vi "Consumer.vi"(8 "error in (no error)":errorcluster, 9 "Data":variant, 10 "Case ID":string, 11 "Monkey in":refnum<class "Monkey.lvclass">) -> (0 "error out":errorcluster, 3 "Monkey out":refnum<class "Monkey.lvclass">)   [LabVIEW 2020, in "Monkey.lvlib" / "Monkey.lvclass"]
uses:
  Monkey.lvclass
  C:/LabVIEW Code/CIRCUS/TALOS/TALOS_PPL.lvlibp/Ancestor/Ancestor/Ancestor.lvclass
  Monkey Consumer Case Selector.ctl
  Analysis Framework/Analysis Framework.lvclass
  Monkey.lvclass/Monkey.ctl
  Run Utilities/TypeDefs/Messages/Schedule Message.ctl
  Run Utilities/TypeDefs/DAQ Control.ctl
  Run Utilities/Schedule/Schedule.lvclass
  Run Utilities/TypeDefs/Script Checker Result.ctl
  Run Utilities/TypeDefs/Messages/Script Checker Message.ctl
  Run Utilities/TypeDefs/Messages/Submit Message.ctl
  Run Utilities/Run Instance/Run Instance.lvclass
  Run Utilities/TypeDefs/Monkey Status.ctl
  Run Utilities/TypeDefs/Messages/Banana Message.ctl
  Run Utilities/TypeDefs/Return Code.ctl
  Inner stop message.ctl
  Run Utilities/Optimiser Cell/Optimiser Cell.lvclass
  C:/LabVIEW Code/CIRCUS/CIRCUS uServices et al/Run Utilities/Cell/Schedule Cell.lvclass
  TALOS/TALOS_PPL.lvlibp/Ancestor/Ancestor/Read ID.vi
  TALOS/TALOS_PPL.lvlibp/Support VIs/Global Constants.vi
  Run Utilities/Run Block/Run Block.lvclass
  TALOS/TALOS_PPL.lvlibp/Father of all uServices/Father of all uServices/Father of all uServices.lvclass
  TALOS/TALOS_PPL.lvlibp
  Run Utilities/Run Utilities.lvlib
  C:/LabVIEW Code/CIRCUS/TALOS/TALOS_PPL.lvlibp/Father of all uServices/Father of all uServices/Father of all uServices.lvclass
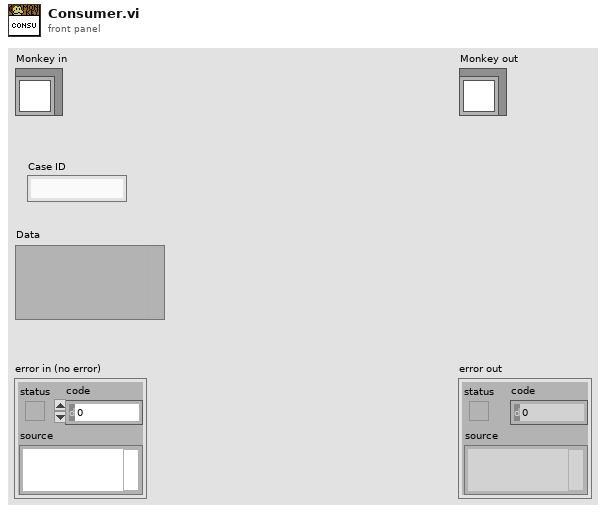
[diagram p1: front panel]
types:
  T1 = typedef "Monkey.lvlib/Monkey.lvclass/Monkey Consumer Case Selector.ctl" = enum16{"Init", "Update GUI", "New schedule", "Check Script", "Submit Script", "Banana arrived", "Optimiser - evaluate RUN", "Optimiser - update RUN", "Quality Check", "What to do next", "Update Crit Lvl", "Skip Run", "Stop Schedule", "Skip schedule", "Append", "Update index", "Delete cell", "Move cell"}
  T2 = cluster{"Font Name:":string, "Size":i16, "Strikeout?":bool, "Italic?":bool, "Underline?":bool, "Outline?":bool, "Shadow?":bool, "Bold?":bool}
  T3 = enum16{"User-specified Font", "Application Font", "System Font", "Dialog Font"}
  T4 = typedef "Run Utilities.lvlib/Schedule Message.ctl" = cluster{"uS Name":string, "Synchronised":bool, "DAQ Control":T5, "Schedule":refnum<class "Schedule.lvclass">, "Append to top?":bool}
  T5 = typedef "Run Utilities.lvlib/DAQ Control.ctl" = enum16{"On", "Off", "External"}
  T6 = typedef "Run Utilities.lvlib/Script Checker Message.ctl" = cluster{"Monkey ID":string, "Script Checker Result":T7}
  T7 = typedef "Run Utilities.lvlib/Script Checker Result.ctl" = enum16{"Passed", "Failed", "Empty"}
  T8 = typedef "Run Utilities.lvlib/Monkey Status.ctl" = enum16{"Init", "Paused", "Ongoing", "Stopped", "Finished (no errors)", "Finished (with errors)"}
  T9 = typedef "Run Utilities.lvlib/Submit Message.ctl" = cluster{"DAQ Control":T5, "Run Instance":refnum<class "Run Instance.lvclass">}
  T10 = typedef "Run Utilities.lvlib/Banana Message.ctl" = cluster{"FPGA Name":string, "Return Code":T11}
  T11 = typedef "Run Utilities.lvlib/Return Code.ctl" = enum16{"All Good", "Retry", "Skip", "Skip All", "ABORT"}
  T12 = cluster{"left":i16, "top":i16, "right":i16, "bottom":i16}
  T13 = typedef "Run Utilities.lvlib/Run Instance.lvclass/Run Instance - GUI.ctl" = cluster{"Script Name":string, "Parameters":string[][], "FPGA Name":string}
  T14 = typedef "Run Utilities.lvlib/Schedule.lvclass/Array of Runs - GUI.ctl" = T15[]
  T15 = typedef "Run Utilities.lvlib/Schedule Cell.lvclass/Cell - GUI.ctl" = cluster{"Background Color":u32, "Number of cycles":u32, "Single RUN":T13, "Quality check":bool, "Cell Type":string}
  T16 = typedef "Monkey.lvlib/Monkey.lvclass/Inner stop message.ctl" = cluster{"Old value":bool, "Gracefully?":bool}
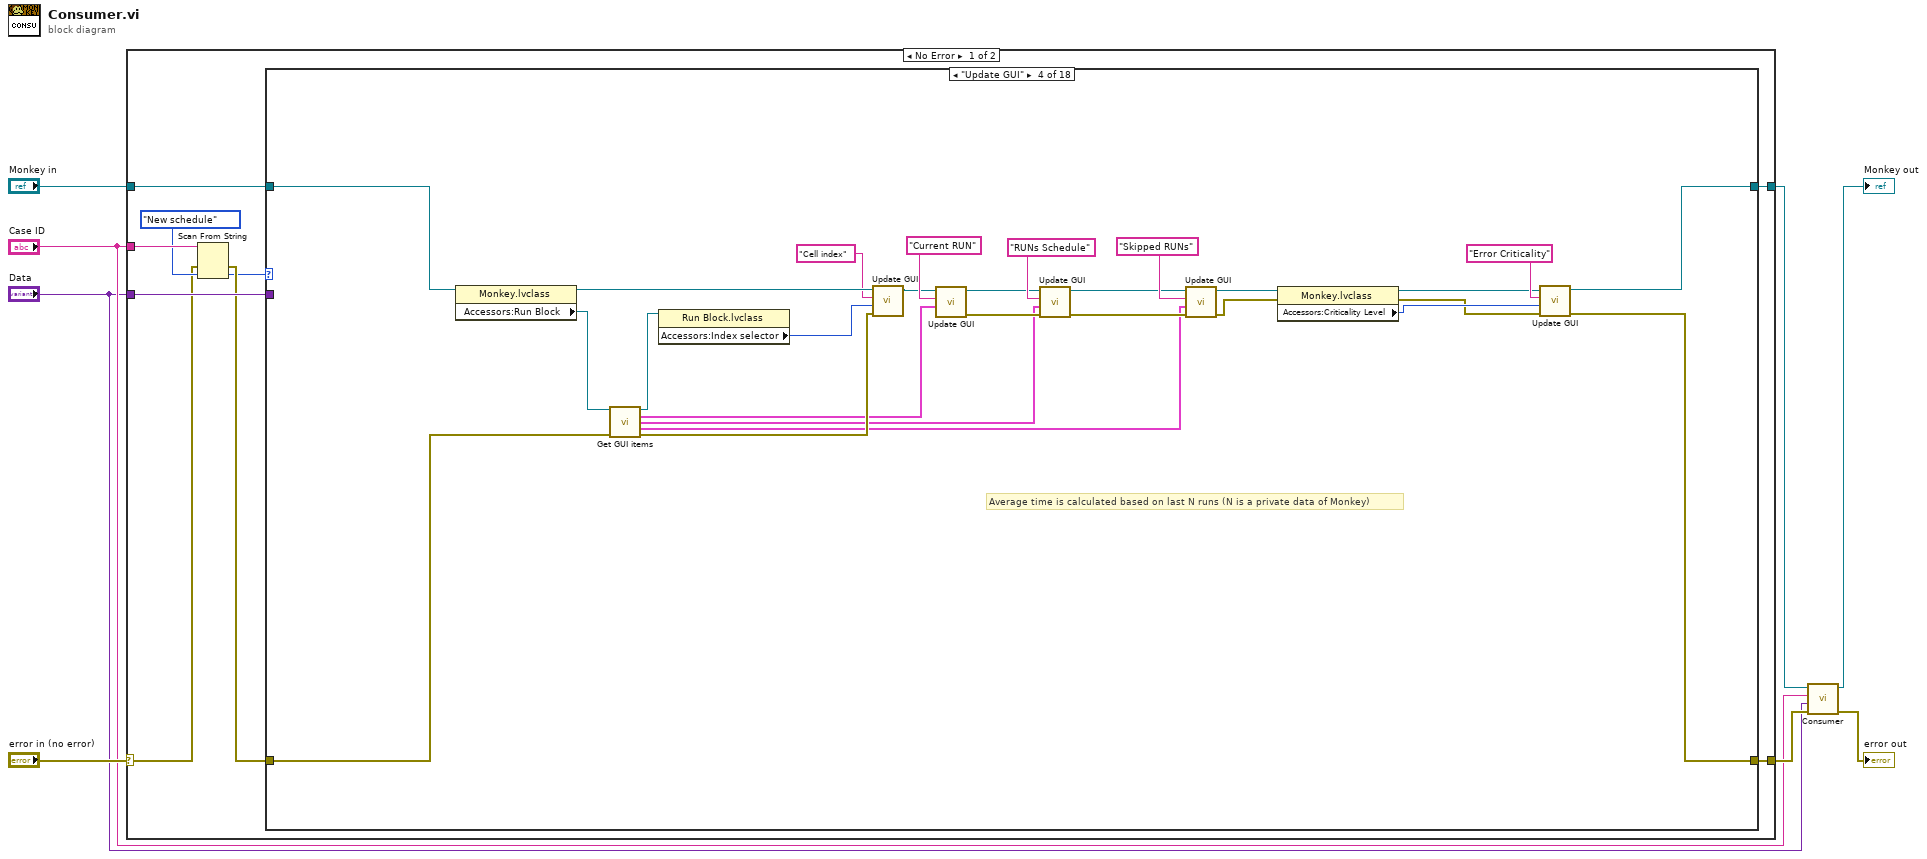
[diagram p0: block diagram]
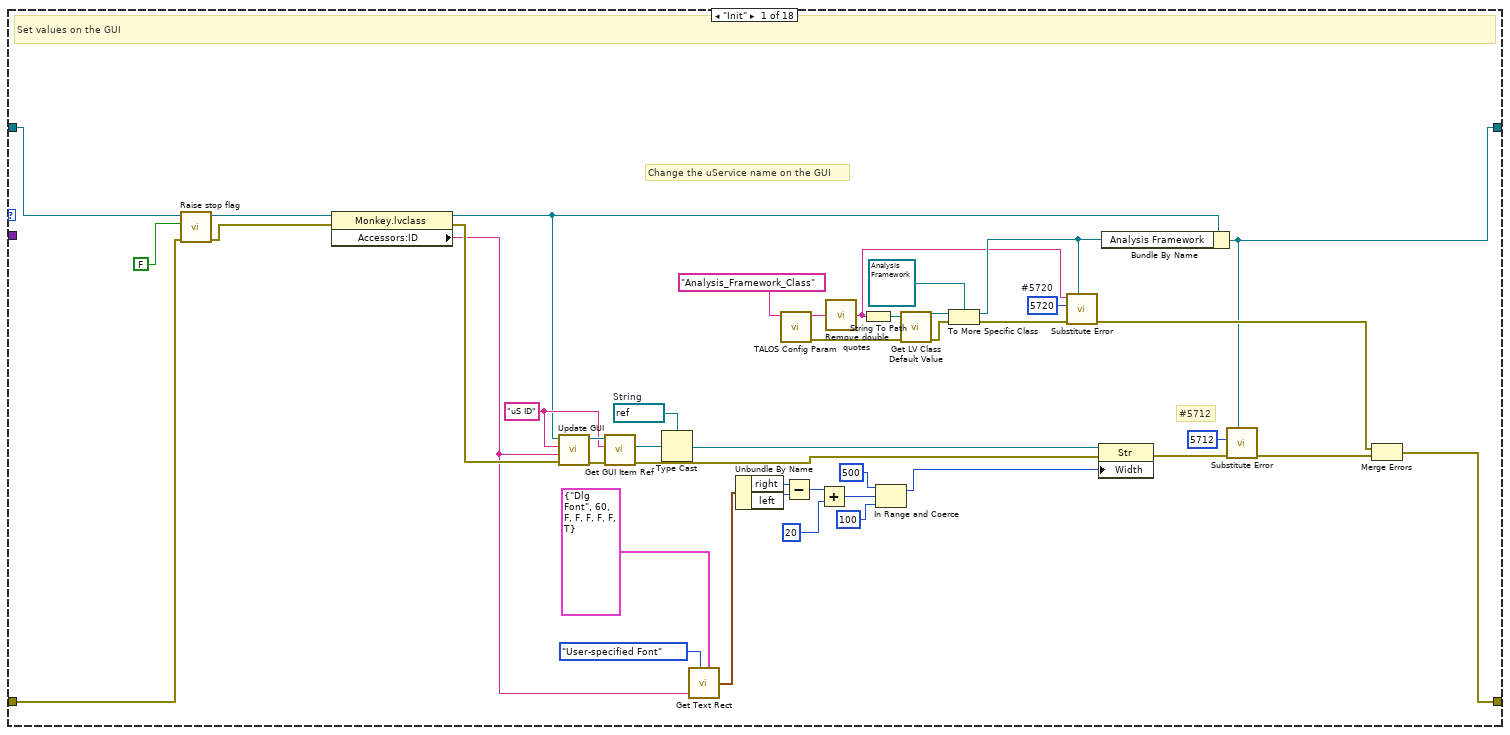
[diagram p2: hidden frame]
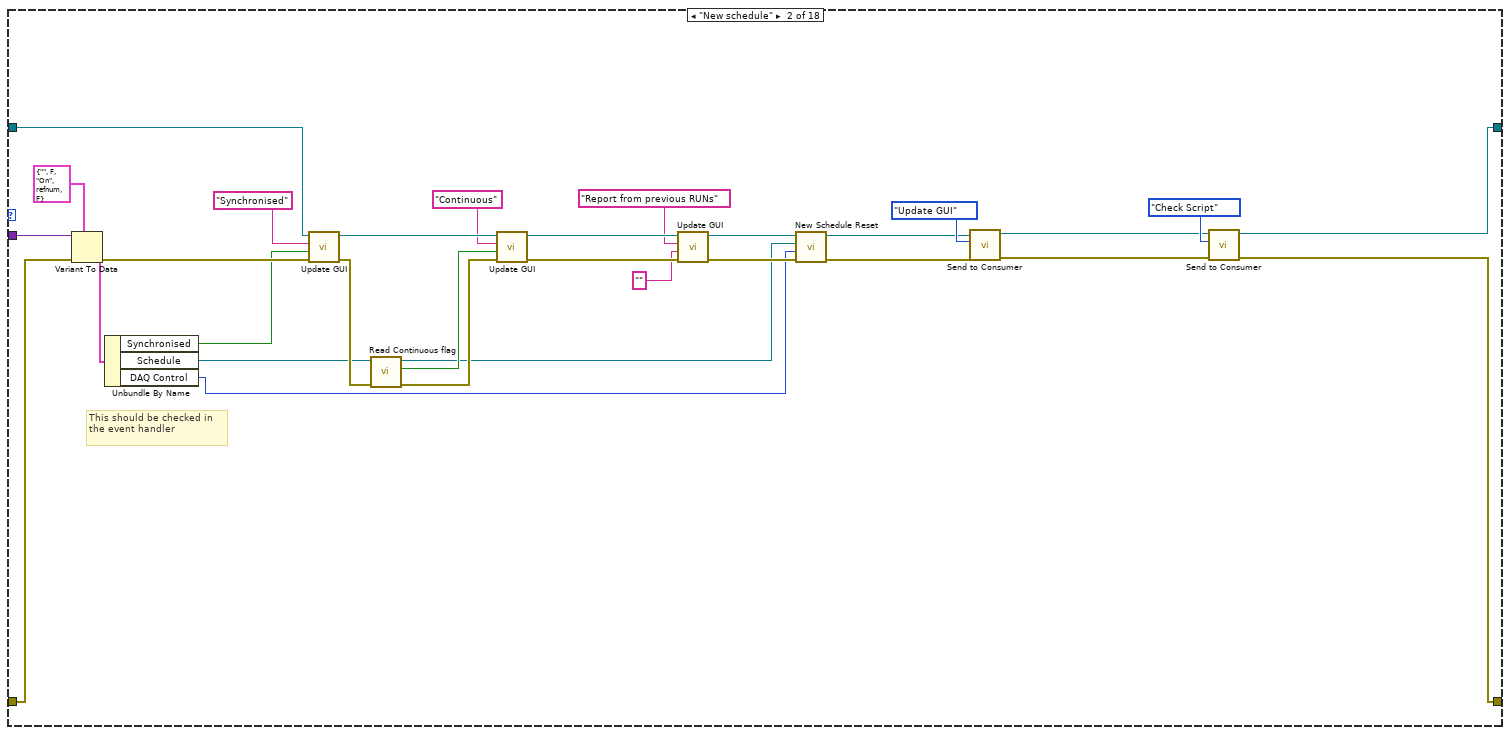
[diagram p3: hidden frame]
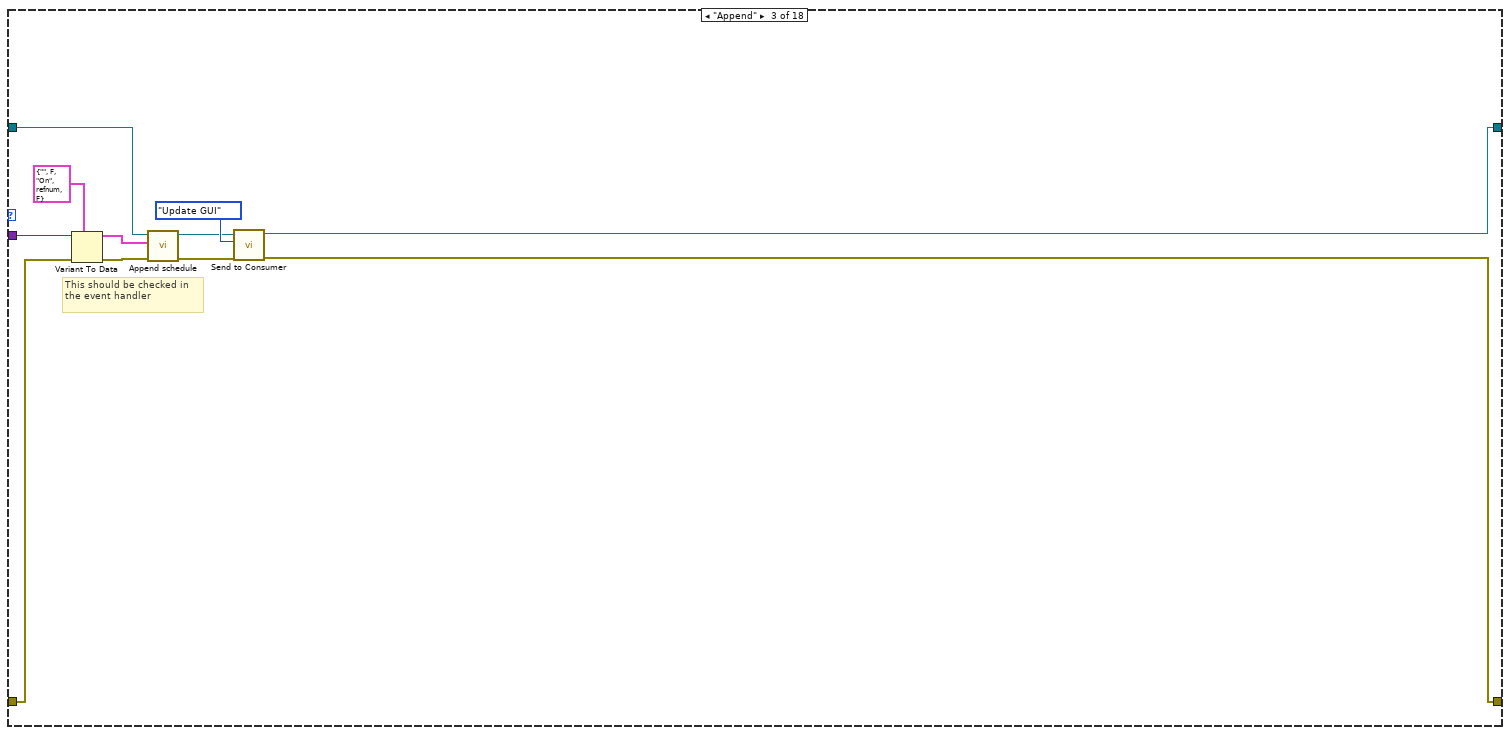
[diagram p4: hidden frame]
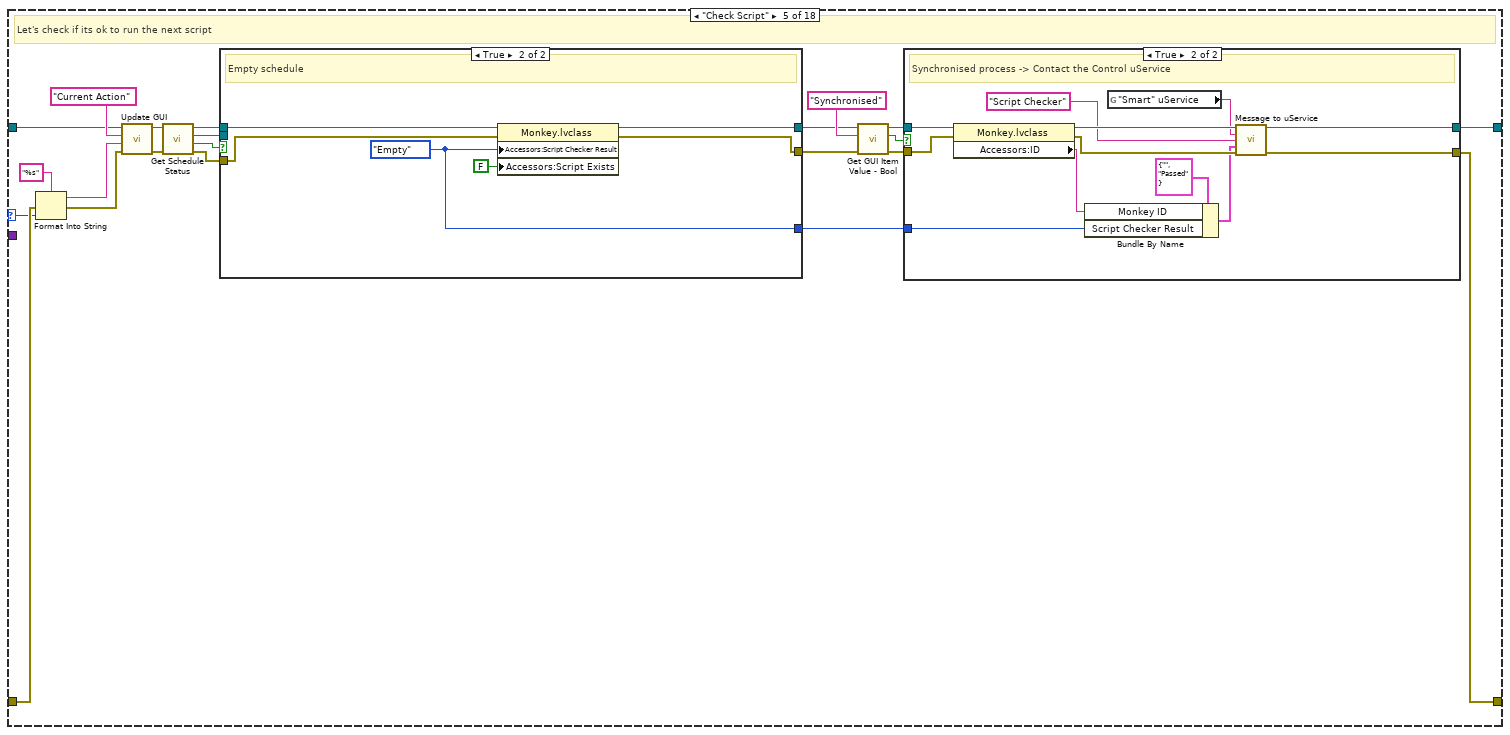
[diagram p5: hidden frame]
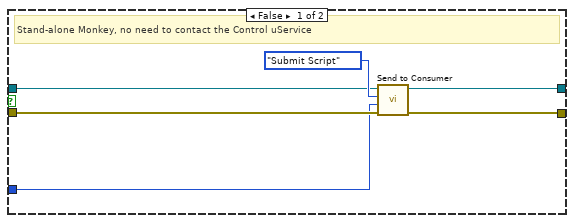
[diagram p6: hidden frame]
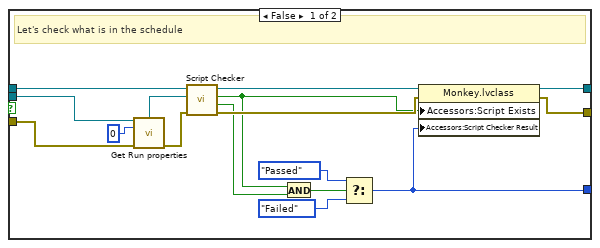
[diagram p7: hidden frame]
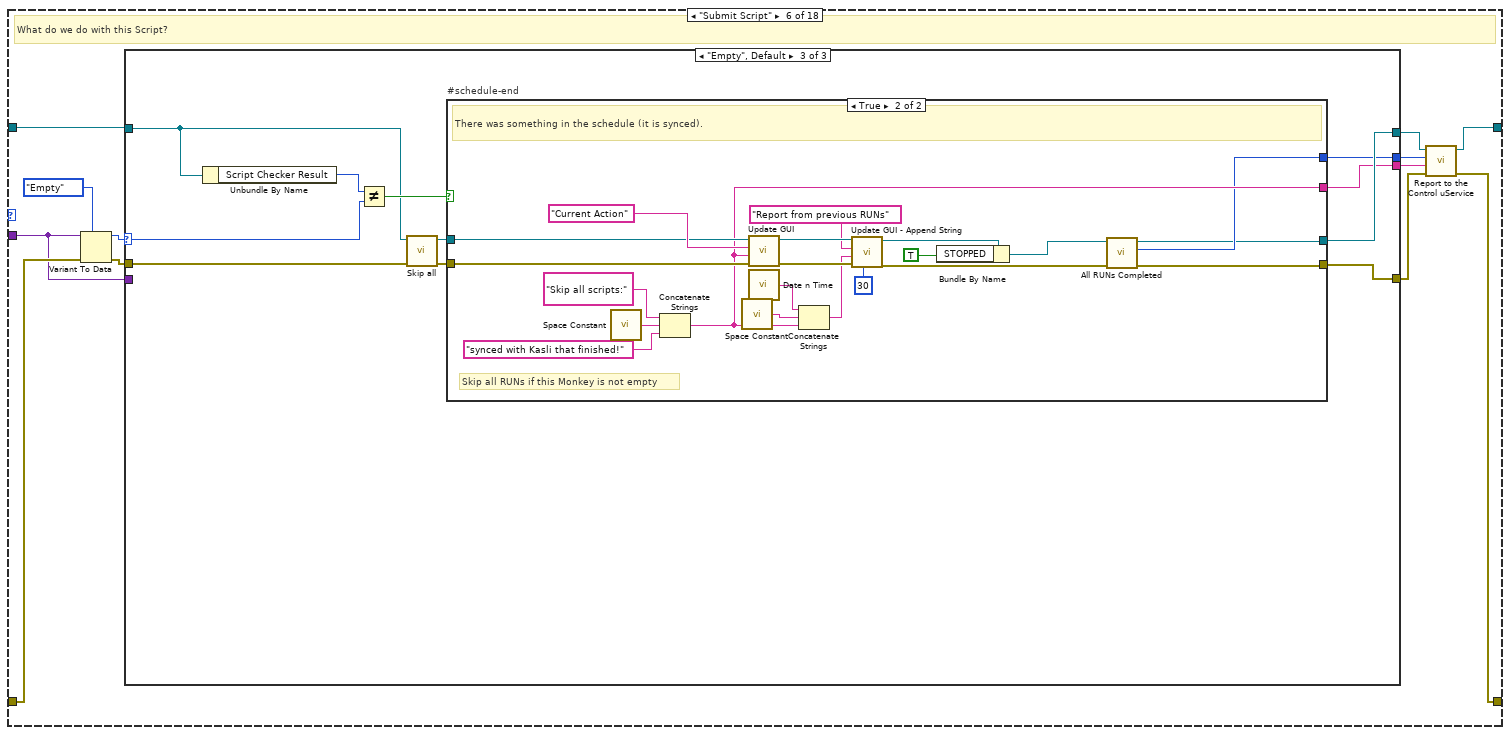
[diagram p8: hidden frame]
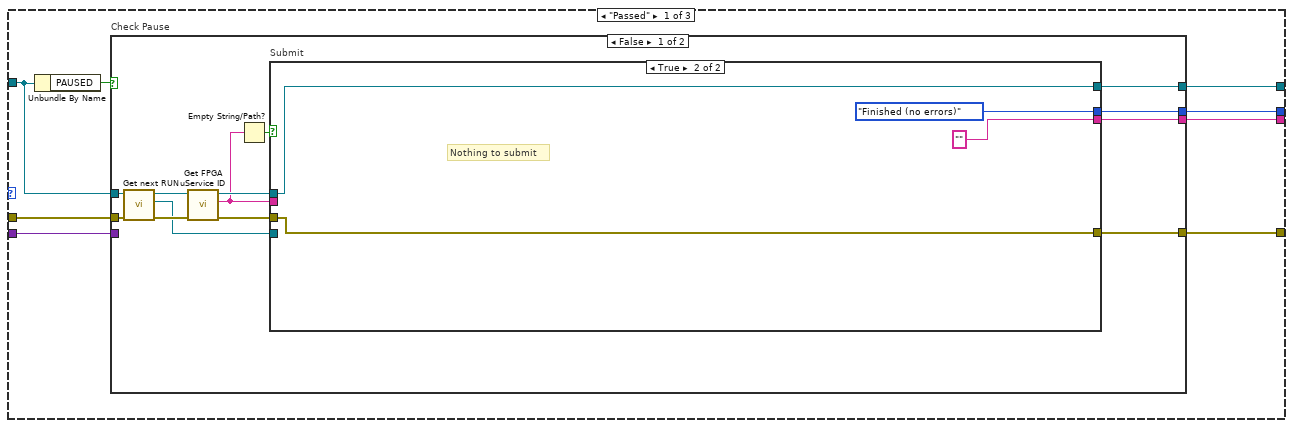
[diagram p9: hidden frame]
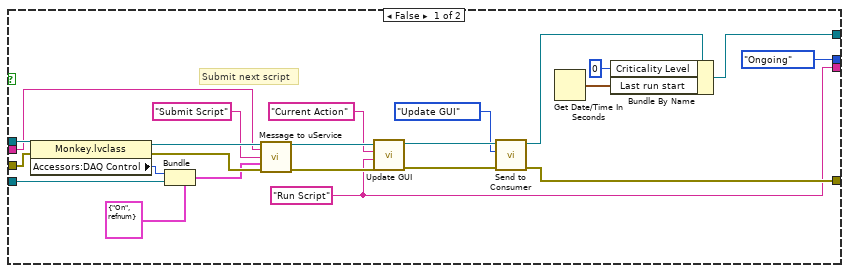
[diagram p10: hidden frame]
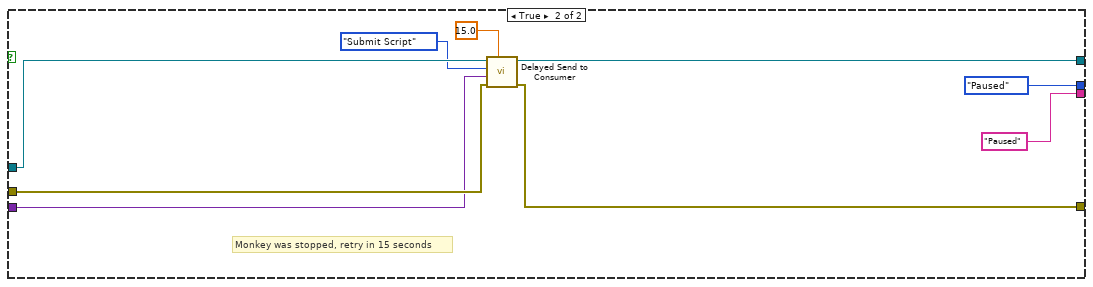
[diagram p11: hidden frame]
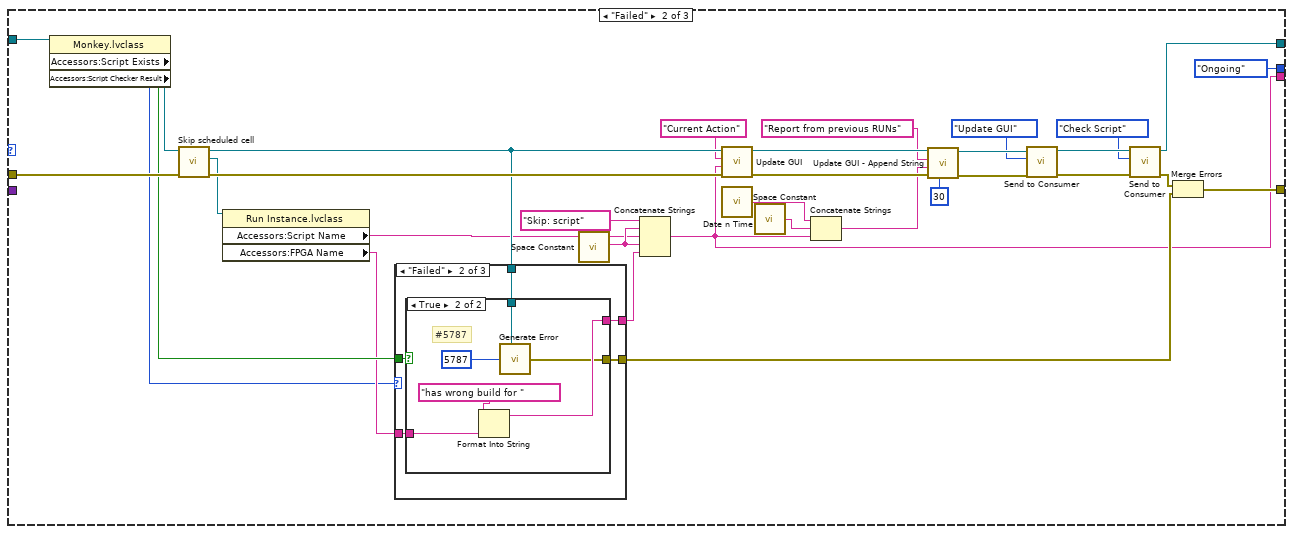
[diagram p12: hidden frame]
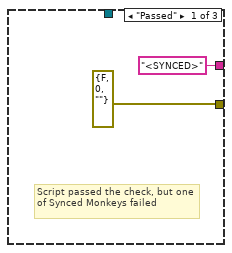
[diagram p13: hidden frame]
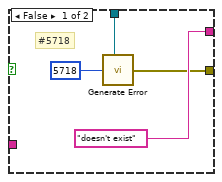
[diagram p14: hidden frame]
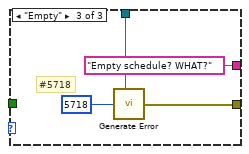
[diagram p15: hidden frame]
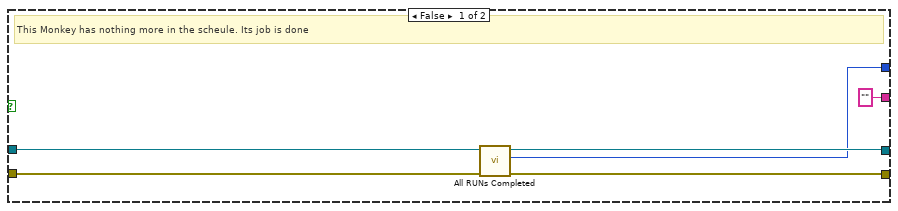
[diagram p16: hidden frame]
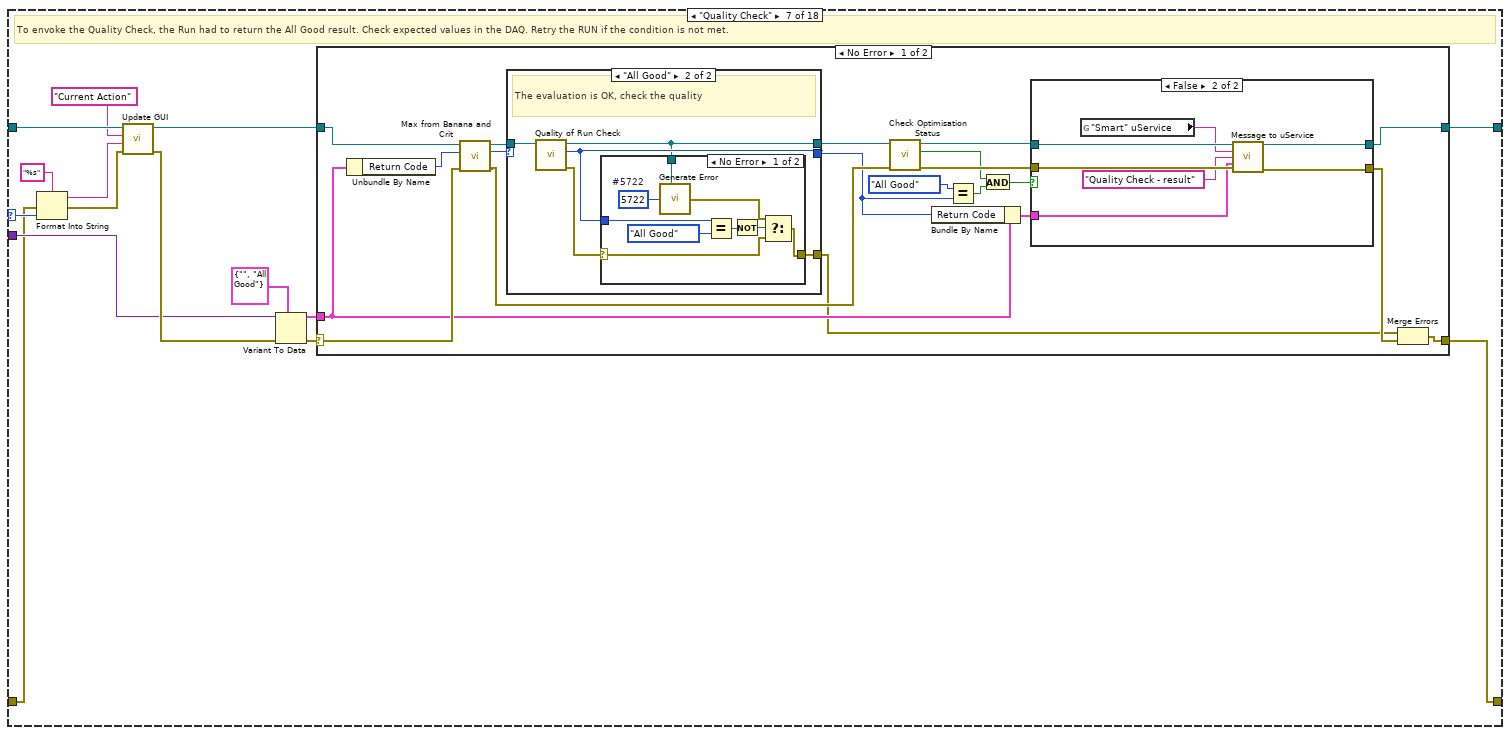
[diagram p17: hidden frame]
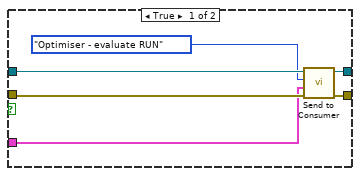
[diagram p18: hidden frame]
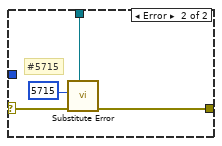
[diagram p20: hidden frame]
diagram:
  n1 = case shown="No Error" "error in (no error)" {
    selector: "error in (no error)" -> [w11 w1022]
    tunnel: [w16 w1023] -> w3
    tunnel: "Monkey in" -> [w17 w1023]
    tunnel: [w14 w1022] -> w6
    tunnel: "Case ID" -> [w13 _]
    tunnel: "Data" -> [w15 _]
    frame No Error {
      n2 = Scan From String(input string=w13, error in=w11, default 1=Monkey_Consumer_Case_Selector."New schedule" ("Consumer Case Selector")) -> (error out=w10:errorcluster, output 1=w9:T1)  [unwired: 2 in, 2 out]
      n3 = case shown="\"Update GUI\"" w9 {
        selector: w9 -> [_ _ _ _ w129 _ w357 _ _ _ _ _ _ _ _ _ _ _]
        tunnel: w17 -> [w25 w78 w94 w125 w131 w202 w365 w446 w538 w613 w642 w860 w895 w935 w989 w994 w1006 w1017]
        tunnel: [w27 w62 w97 w119 w140 w196 w363 w444 w535 w615 w644 w870 w898 w944 w979 w997 w1002 w1013] -> w16
        tunnel: w15 -> [_ w87 w101 _ _ w191 w364 w443 w534 w611 w646 w875 w899 w945 _ w1001 _ w1012]
        tunnel: [w30 w61 w96 w118 w139 w194 w352 w445 w536 w614 w643 w869 w897 w943 w980 w995 w1004 w1015] -> w14
        tunnel: w10 -> [w23 w84 w99 w105 w133 w201 w354 w447 w537 w612 w645 w874 w905 w947 w988 w991 w1005 w1016]
        frame "Init" {
          w32 = 5720  # #5720
          w55 = refnum<vi> refnum  # String
          w58 = "uS ID" ("GUI Item Name")
          # "Change the uService name on the GUI"
          # "#5712"
          # "Set values on the GUI"
          n4 = call-dynamic "Raise stop flag.vi"("error in (no error)"=w23, "on/off"=FALSE ("value"), "Monkey in"=w25) -> ("error out"=w24:errorcluster, "Monkey out"=w26:refnum<class "Monkey.lvclass">)  [unwired: 7 in]
          n5 = property class="Monkey.lvclass"(reference=w26, error in=w24) -> (reference out=w28:refnum<class "Monkey.lvclass">, error out=w53:errorcluster, "Accessors:ID"=w47:string)
          n6 = call "Update GUI.vi"("error in (no error)"=w53, "Data"=w47, "GUI Item Name"=w58, "uService Template in"=w28) -> ("error out"=w57:errorcluster, "uService Template out"=w59:refnum<class "Monkey.lvclass">)  [unwired: 6 in]
          n7 = call "Get GUI Item Ref.vi"("error in (no error)"=w57, "FP Item Name"=w58, "uService Template in"=w59) -> ("error out"=w51:errorcluster, "Ctl Refnum"=w56:refnum<vi>)  [unwired: 6 in, 1 out]
          n8 = Type Cast(type=w55, x=w56) -> (*(type *) &x=w52:refnum<vi>)
          n9 = call <vilib>:"Get Text Rect.vi"("desired font(Application)"=T3."User-specified Font", "text"=w47, "[user-specified font]"=T2 {"Font Name:"="Dlg Font", "Size"=60, "Strikeout?"=FALSE, "Italic?"=FALSE, "Underline?"=FALSE, "Outline?"=FALSE, "Shadow?"=FALSE, "Bold?"=TRUE}) -> ("rect"=w48:T12)  [unwired: 6 in]
          n10 = Unbundle By Name(w48) -> ("right"=w46:i16, "left"=w45:i16)
          n11 = call "TALOS Config Param.vi"("Parameter Name"="Analysis_Framework_Class") -> ("error out"=w20:errorcluster, "Output"=w19:string)  [unwired: 9 in]
          n12 = Subtract(x=w46, y=w45) -> (x-y=w44:i16)
          n13 = Add(x=w44, y=i16 20) -> (x+y=w41:i16)
          n14 = call "Remove double quotes.vi"("Input string"=w19) -> ("Output string"=w21:string)  [unwired: 4 in]
          n15 = String To Path(string=w21) -> (path=w37:path)
          n16 = In Range and Coerce(upper limit=i16 500, x=w41, lower limit=i16 100) -> (coerced(x)=w38:i16)  [unwired: 1 out]
          n17 = call <vilib>:"Get LV Class Default Value.vi"("error in (no error)"=w20, "class path"=w37) -> ("error out"=w36:errorcluster, "object"=w35:refnum<class>)  [unwired: 8 in]
          n18 = To More Specific Class(target class=refnum<class "Analysis Framework.lvclass"> refnum ("Analysis Framework"), reference=w35, error in=w36) -> (specific class reference=w29:refnum<class "Analysis Framework.lvclass">, error out=w33:errorcluster)
          n19 = call "Substitute Error.vi"("LabVIEW Object"=w29, "error in (no error)"=w33, "Error Code"=w32, "Optional String"=w21) -> ("error out"=w60:errorcluster)  [unwired: 7 in]
          n20 = property class="Str"(reference=w52, error in=w51, "Width"=w38) -> (error out=w42:errorcluster)  [unwired: 1 out]
          n21 = Bundle By Name(cluster=w28, "Analysis Framework"=w29) -> (w27:refnum<class "Monkey.lvclass">)
          n22 = call "Substitute Error.vi"("LabVIEW Object"=w27, "error in (no error)"=w42, "Error Code"=5712) -> ("error out"=w31:errorcluster)  [unwired: 8 in]
          n23 = Merge Errors(w60, w31) -> (w30:errorcluster)
        }
        frame "New schedule" {
          # "This should be checked in the event handler"
          n24 = Variant To Data(error in=w84, type=T4 {"uS Name"="", "Synchronised"=FALSE, "DAQ Control"=enum."On", "Schedule"=refnum, "Append to top?"=FALSE} ("Monkey Schedule Message"), Variant=w87) -> (data=w85:T4, error out=w90:errorcluster)
          n25 = Unbundle By Name(w85) -> ("Synchronised"=w79:bool, "Schedule"=w72:refnum<class "Schedule.lvclass">, "DAQ Control"=w64:T5)
          n26 = call "Update GUI.vi"("error in (no error)"=w90, "Data"=w79, "GUI Item Name"="Synchronised", "uService Template in"=w78) -> ("error out"=w73:errorcluster, "uService Template out"=w82:refnum<class "Monkey.lvclass">)  [unwired: 6 in]
          n27 = call-dynamic "Read Continuous flag.vi"("error in (no error)"=w73, "Schedule in"=w72) -> ("error out"=w88:errorcluster, "Continuous flag"=w81:bool, "Schedule out"=w65:refnum<class "Schedule.lvclass">)  [unwired: 7 in]
          n28 = call "Update GUI.vi"("error in (no error)"=w88, "Data"=w81, "GUI Item Name"="Continuous", "uService Template in"=w82) -> ("error out"=w77:errorcluster, "uService Template out"=w76:refnum<class "Monkey.lvclass">)  [unwired: 6 in]
          n29 = call "Update GUI.vi"("error in (no error)"=w77, "Data"="", "GUI Item Name"="Report from previous RUNs", "uService Template in"=w76) -> ("error out"=w89:errorcluster, "uService Template out"=w67:refnum<class "Monkey.lvclass">)  [unwired: 6 in]
          n30 = call-dynamic "New Schedule Reset.vi"("error in (no error)"=w89, "DAQ Control"=w64, "Schedule"=w65, "Monkey in"=w67) -> ("error out"=w63:errorcluster, "Monkey out"=w66:refnum<class "Monkey.lvclass">)  [unwired: 6 in]
          n31 = call "Send to Consumer.vi"("error in (no error)"=w63, "Case ID"=Monkey_Consumer_Case_Selector."Update GUI" ("Monkey Consumer Case Selector"), "uService Template in"=w66) -> ("error out"=w68:errorcluster, "uService Template out"=w69:refnum<class "Monkey.lvclass">)  [unwired: 7 in]
          n32 = call "Send to Consumer.vi"("error in (no error)"=w68, "Case ID"=Monkey_Consumer_Case_Selector."Check Script" ("Monkey Consumer Case Selector"), "uService Template in"=w69) -> ("error out"=w61:errorcluster, "uService Template out"=w62:refnum<class "Monkey.lvclass">)  [unwired: 7 in]
        }
        frame "Append" {
          # "This should be checked in the event handler"
          n33 = Variant To Data(error in=w99, type=T4 {"uS Name"="", "Synchronised"=FALSE, "DAQ Control"=enum."On", "Schedule"=refnum, "Append to top?"=FALSE} ("Monkey Schedule Message"), Variant=w101) -> (data=w95:T4, error out=w91:errorcluster)
          n34 = call-dynamic "Append schedule.vi"("error in (no error)"=w91, "Monkey Schedule Message"=w95, "Monkey in"=w94) -> ("error out"=w92:errorcluster, "Monkey out"=w93:refnum<class "Monkey.lvclass">)  [unwired: 7 in]
          n35 = call "Send to Consumer.vi"("error in (no error)"=w92, "Case ID"=Monkey_Consumer_Case_Selector."Update GUI" ("Monkey Consumer Case Selector"), "uService Template in"=w93) -> ("error out"=w96:errorcluster, "uService Template out"=w97:refnum<class "Monkey.lvclass">)  [unwired: 7 in]
        }
        frame "Update GUI" {
          # "Average time is calculated based on last N runs (N is a private data of Monkey)"
          n36 = property class="Monkey.lvclass"(reference=w125) -> (reference out=w108:refnum<class "Monkey.lvclass">, "Accessors:Run Block"=w104:refnum<class "Run Block.lvclass">)  [unwired: 1 in, 1 out]
          n37 = call-dynamic "Get GUI items.vi"("Run Block in"=w104, "error in (no error)"=w105) -> ("Run Block out"=w103:refnum<class "Run Block.lvclass">, "Current RUN"=w120:T13, "Schedule"=w109:T14, "Skipped RUNs"=w122:T14, "error out"=w128:errorcluster)  [unwired: 9 in]
          n38 = property class="Run Block.lvclass"(reference=w103) -> ("Accessors:Index selector"=w102:i32)  [unwired: 1 in, 2 out]
          n39 = call "Update GUI.vi"("error in (no error)"=w128, "Data"=w102, "GUI Item Name"="Cell index", "uService Template in"=w108) -> ("uService Template out"=w107:refnum<class "Monkey.lvclass">)  [unwired: 6 in, 1 out]
          n40 = call "Update GUI.vi"("Data"=w120, "GUI Item Name"="Current RUN", "uService Template in"=w107) -> ("error out"=w110:errorcluster, "uService Template out"=w111:refnum<class "Monkey.lvclass">)  [unwired: 7 in]
          n41 = call "Update GUI.vi"("error in (no error)"=w110, "Data"=w109, "GUI Item Name"="RUNs Schedule", "uService Template in"=w111) -> ("error out"=w127:errorcluster, "uService Template out"=w123:refnum<class "Monkey.lvclass">)  [unwired: 6 in]
          n42 = call "Update GUI.vi"("error in (no error)"=w127, "Data"=w122, "GUI Item Name"="Skipped RUNs", "uService Template in"=w123) -> ("error out"=w114:errorcluster, "uService Template out"=w115:refnum<class "Monkey.lvclass">)  [unwired: 6 in]
          n43 = property class="Monkey.lvclass"(reference=w115, error in=w114) -> (reference out=w113:refnum<class "Monkey.lvclass">, error out=w112:errorcluster, "Accessors:Criticality Level"=w116:u8)
          n44 = call "Update GUI.vi"("error in (no error)"=w112, "Data"=w116, "GUI Item Name"="Error Criticality", "uService Template in"=w113) -> ("error out"=w118:errorcluster, "uService Template out"=w119:refnum<class "Monkey.lvclass">)  [unwired: 6 in]
        }
        frame "Check Script" {
          # "Let's check if its ok to run the next script"
          n45 = Format Into String(format string="%s", error in=w133, w129) -> (resulting string=w136:string, error out=w134:errorcluster)  [unwired: 1 in]
          n46 = call "Update GUI.vi"("error in (no error)"=w134, "Data"=w136, "GUI Item Name"="Current Action", "uService Template in"=w131) -> ("error out"=w132:errorcluster, "uService Template out"=w130:refnum<class "Monkey.lvclass">)  [unwired: 6 in]
          n47 = call-dynamic "Get Schedule Status.vi"("error in (no error)"=w132, "Monkey in"=w130) -> ("error out"=w150:errorcluster, "Empty?"=w149:bool, "Schedule out"=w148:refnum<class "Schedule.lvclass">, "Monkey out"=w138:refnum<class "Monkey.lvclass">)  [unwired: 6 in]
          n48 = case shown="True" w149 {
            tunnel: w138 -> [w179 w190]
            tunnel: w150 -> [w182 w187]
            tunnel: w148 -> [w181 _]
            tunnel: [w173 w189] -> w146
            tunnel: [w172 w186] -> w143
            tunnel: [w170 w185] -> w141
            frame False {
              # "Let's check what is in the schedule"
              n49 = call "Get Run properties.vi"("Schedule in"=w181, "index"=0, "error in (no error)"=w182) -> ("Run Instance"=w169:refnum<class "Run Instance.lvclass">, "error out"=w183:errorcluster)  [unwired: 5 in, 6 out]
              n50 = call "Script Checker.vi"("error in (no error)"=w183, "Run"=w169, "Monkey in"=w179) -> ("error out"=w184:errorcluster, "Correct Build?"=w177:bool, "Script exists?"=w171:bool, "Monkey out"=w178:refnum<class "Monkey.lvclass">)  [unwired: 5 in]
              n51 = And(x=w171, y=w177) -> (x .and. y?=w174:bool)
              n52 = Select(t=Script_Checker_Result."Passed" ("Script Checker Result"), s=w174, f=Script_Checker_Result."Failed" ("Script Checker Result")) -> (s? t:f=w170:T7)
              n53 = property class="Monkey.lvclass"(reference=w178, error in=w184, "Accessors:Script Exists"=w171, "Accessors:Script Checker Result"=w170) -> (reference out=w173:refnum<class "Monkey.lvclass">, error out=w172:errorcluster)
            }
            frame True {
              w185 = Script_Checker_Result."Empty" ("Script Checker Result")
              # "Empty schedule"
              n54 = property class="Monkey.lvclass"(reference=w190, error in=w187, "Accessors:Script Checker Result"=w185, "Accessors:Script Exists"=FALSE ("Script Exists")) -> (reference out=w189:refnum<class "Monkey.lvclass">, error out=w186:errorcluster)
            }
          }
          n55 = call "Get GUI Item Value - Bool.vi"("error in (no error)"=w143, "FP Item Name"="Synchronised", "uService Template in"=w146) -> ("error out"=w142:errorcluster, "Value"=w144:bool, "uService Template out"=w145:refnum<class "Monkey.lvclass">)  [unwired: 6 in]
          n56 = case shown="True" w144 {
            tunnel: w145 -> [w154 w168]
            tunnel: w142 -> [w156 w165]
            tunnel: w141 -> [w151 w160]
            tunnel: [w153 w159] -> w140
            tunnel: [w152 w158] -> w139
            frame False {
              # "Stand-alone Monkey, no need to contact the Control uService"
              n57 = call "Send to Consumer.vi"("error in (no error)"=w156, "Data"=w151, "Case ID"=Monkey_Consumer_Case_Selector."Submit Script" ("Monkey Consumer Case Selector"), "uService Template in"=w154) -> ("error out"=w152:errorcluster, "uService Template out"=w153:refnum<class "Monkey.lvclass">)  [unwired: 6 in]
            }
            frame True {
              # "Synchronised process -> Contact the Control uService"
              n58 = property class="Monkey.lvclass"(reference=w168, error in=w165) -> (reference out=w167:refnum<class "Monkey.lvclass">, error out=w166:errorcluster, "Accessors:ID"=w163:string)
              n59 = Bundle By Name(cluster=T6 {"Monkey ID"="", "Script Checker Result"=enum."Passed"} ("Message"), "Monkey ID"=w163, "Script Checker Result"=w160) -> (w162:T6)
              n60 = global read "Global Constants.vi" "\"Smart\" uService"() -> (w157:string)
              n61 = call "Message to uService.vi"("Father of all uServices in"=w167, "uService ID"=w157, "Message"="Script Checker", "Data"=w162, "error in (no error)"=w166) -> ("Father of all uServices out"=w159:refnum<class "Monkey.lvclass">, "error out"=w158:errorcluster)  [unwired: 9 in]
            }
          }
        }
        frame "Submit Script" {
          # "What do we do with this Script?"
          n62 = Variant To Data(error in=w201, type=Script_Checker_Result."Empty" ("Script Checker Result"), Variant=w191) -> (data=w198:T7, error out=w200:errorcluster)
          n63 = case shown="\"Empty\", Default" w198 {
            selector: w198 -> [_ _ w323]
            tunnel: w202 -> [w205 w272 w319]
            tunnel: w200 -> [w206 w271 w318]
            tunnel: [w209 w270 w317] -> w197
            tunnel: [w210 w269 w316] -> w195
            tunnel: [w208 Monkey_Status."Ongoing" ("Monkey Status") w315] -> w193
            tunnel: [w207 w260 w314] -> w192
            tunnel: w191 -> [w203 _ _]
            frame "Passed" {
              n64 = Unbundle By Name(w205) -> ("PAUSED"=w204:bool)
              n65 = case "Check Pause" shown="False" w204 {
                tunnel: [w221 w254] -> w210
                tunnel: [w220 w256] -> w209
                tunnel: [w219 Monkey_Status."Paused" ("Monkey Status")] -> w208
                tunnel: [w218 "Paused"] -> w207
                tunnel: w206 -> [w214 w255]
                tunnel: w205 -> [w211 w257]
                tunnel: w203 -> [_ w252]
                frame False {
                  n66 = call "Get next RUN.vi"("error in (no error)"=w214, "Monkey in"=w211) -> ("error out"=w223:errorcluster, "Current RUN"=w222:refnum<class "Run Instance.lvclass">, "Monkey out"=w217:refnum<class "Monkey.lvclass">)  [unwired: 7 in]
                  n67 = call-dynamic "Get FPGA uService ID.vi"("error in (no error)"=w223, "Monkey in"=w217) -> ("error out"=w215:errorcluster, "FPGA uService ID"=w212:string, "Monkey out"=w216:refnum<class "Monkey.lvclass">)  [unwired: 7 in]
                  n68 = Empty String/Path?(string/path=w212) -> (empty?=w213:bool)
                  n69 = case "Submit" shown="True" w213 {
                    tunnel: w222 -> [w243 _]
                    tunnel: [w235 w249] -> w221
                    tunnel: [w230 w250] -> w220
                    tunnel: [Monkey_Status."Ongoing" ("Monkey Status") Monkey_Status."Finished (no errors)" ("Monkey Status")] -> w219
                    tunnel: [w228 ""] -> w218
                    tunnel: w216 -> [w226 w250]
                    tunnel: w215 -> [w225 w249]
                    tunnel: w212 -> [w224 _]
                    frame False {
                      w228 = "Run Script"
                      # "Submit next script"
                      n70 = property class="Monkey.lvclass"(reference=w226, error in=w225) -> (reference out=w242:refnum<class "Monkey.lvclass">, error out=w245:errorcluster, "Accessors:DAQ Control"=w241:T5)
                      n71 = Bundle(cluster=T9 {"DAQ Control"=enum."On", "Run Instance"=refnum} ("Submit Msg"), "DAQ Control"=w241, "Run Instance"=w243) -> (w240:T9)
                      n72 = call "Message to uService.vi"("Father of all uServices in"=w242, "uService ID"=w224, "Message"="Submit Script", "Data"=w240, "error in (no error)"=w245) -> ("Father of all uServices out"=w239:refnum<class "Monkey.lvclass">, "error out"=w238:errorcluster)  [unwired: 9 in]
                      n73 = call "Update GUI.vi"("error in (no error)"=w238, "Data"=w228, "GUI Item Name"="Current Action", "uService Template in"=w239) -> ("error out"=w236:errorcluster, "uService Template out"=w246:refnum<class "Monkey.lvclass">)  [unwired: 6 in]
                      n74 = call "Send to Consumer.vi"("error in (no error)"=w236, "Case ID"=Monkey_Consumer_Case_Selector."Update GUI" ("Monkey Consumer Case Selector"), "uService Template in"=w246) -> ("error out"=w235:errorcluster, "uService Template out"=w233:refnum<class "Monkey.lvclass">)  [unwired: 7 in]
                      n75 = Get Date/Time In Seconds() -> (seconds since 1Jan1904=w231:timestamp)
                      n76 = Bundle By Name(cluster=w233, "Criticality Level"=u8 0, "Last run start"=w231) -> (w230:refnum<class "Monkey.lvclass">)
                    }
                    frame True {
                      # "Nothing to submit"
                    }
                  }
                }
                frame True {
                  # "Monkey was stopped, retry in 15 seconds"
                  n77 = call "Delayed Send to Consumer.vi"("Seconds (5)"=15.0, "error in (no error)"=w255, "Data"=w252, "Case ID"=Monkey_Consumer_Case_Selector."Submit Script" ("Monkey Consumer Case Selector"), "Father of all uServices in"=w257) -> ("error out"=w254:errorcluster, "Father of all uServices out"=w256:refnum<class "Monkey.lvclass">)  [unwired: 5 in]
                }
              }
            }
            frame "Failed" {
              n78 = property class="Monkey.lvclass"(reference=w272) -> (reference out=w267:refnum<class "Monkey.lvclass">, "Accessors:Script Exists"=w268:bool, "Accessors:Script Checker Result"=w262:T7)  [unwired: 1 in, 1 out]
              n79 = call-dynamic "Skip scheduled cell.vi"("error in (no error)"=w271, "Monkey in"=w267) -> ("error out"=w292:errorcluster, "Skipped Run"=w266:refnum<class "Run Instance.lvclass">, "Monkey out"=w291:refnum<class "Monkey.lvclass">)  [unwired: 7 in]
              n80 = property class="Run Instance.lvclass"(reference=w266) -> ("Accessors:Script Name"=w265:string, "Accessors:FPGA Name"=w264:string)  [unwired: 1 in, 2 out]
              n81 = case shown="\"Failed\"" w262 {
                tunnel: ["<SYNCED>" w299 "Empty schedule? WHAT?"] -> w275
                tunnel: [errorcluster {"status"=FALSE, "code"=0, "source"=""} ("error out") w298 w311] -> w274
                tunnel: w268 -> [_ w297 _]
                tunnel: w264 -> [_ w296 _]
                tunnel: w291 -> [_ w295 w310]
                frame "Passed" {
                  # "Script passed the check, but one of Synced Monkeys failed"
                }
                frame "Failed" {
                  n82 = case shown="True" w297 {
                    tunnel: w296 -> [_ w309]
                    tunnel: w295 -> [w302 w306]
                    tunnel: ["doesn't exist" w305] -> w299
                    tunnel: [w300 w304] -> w298
                    frame False {
                      # "#5718"
                      n83 = call "Generate Error.vi"("Class"=w302, "Error Code"=5718) -> ("error out"=w300:errorcluster)  [unwired: 5 in]
                    }
                    frame True {
                      # "#5787"
                      n84 = Format Into String(initial string="has wrong build for " ("t"), w309) -> (resulting string=w305:string)  [unwired: 2 in, 1 out]
                      n85 = call "Generate Error.vi"("Class"=w306, "Error Code"=5787) -> ("error out"=w304:errorcluster)  [unwired: 5 in]
                    }
                  }
                }
                frame "Empty" {
                  # "#5718"
                  n86 = call "Generate Error.vi"("Class"=w310, "Error Code"=5718) -> ("error out"=w311:errorcluster)  [unwired: 5 in]
                }
              }
              n87 = call <vilib>:"Space Constant.vi"() -> ("String"=w281:string)
              n88 = Concatenate Strings("Skip: script" ("GUI Item Name"), w281, w265, w281, w275) -> (w260:string)
              n89 = call "Update GUI.vi"("error in (no error)"=w292, "Data"=w260, "GUI Item Name"="Current Action", "uService Template in"=w291) -> ("error out"=w286:errorcluster, "uService Template out"=w287:refnum<class "Monkey.lvclass">)  [unwired: 6 in]
              n90 = call "Date n Time.vi"() -> ("Date & Time"=w277:string)  [unwired: 5 in]
              n91 = call <vilib>:"Space Constant.vi"() -> ("String"=w278:string)
              n92 = Concatenate Strings(w277, w278, w260) -> (w276:string)
              n93 = call "Update GUI - Append String.vi"("Lines to keep"=u8 30, "error in (no error)"=w286, "String"=w276, "GUI Item Name"="Report from previous RUNs", "Father of all uServices in"=w287) -> ("error out"=w288:errorcluster, "Father of all uServices out"=w290:refnum<class "Monkey.lvclass">)  [unwired: 5 in]
              n94 = call "Send to Consumer.vi"("error in (no error)"=w288, "Case ID"=Monkey_Consumer_Case_Selector."Update GUI" ("Monkey Consumer Case Selector"), "uService Template in"=w290) -> ("error out"=w283:errorcluster, "uService Template out"=w289:refnum<class "Monkey.lvclass">)  [unwired: 7 in]
              n95 = call "Send to Consumer.vi"("error in (no error)"=w283, "Case ID"=Monkey_Consumer_Case_Selector."Check Script" ("Monkey Consumer Case Selector"), "uService Template in"=w289) -> ("error out"=w273:errorcluster, "uService Template out"=w270:refnum<class "Monkey.lvclass">)  [unwired: 7 in]
              n96 = Merge Errors(w273, w274) -> (w269:errorcluster)
            }
            frame "Empty", Default {
              n97 = Unbundle By Name(w319) -> ("Script Checker Result"=w324:T7)
              n98 = Not Equal?(x=w324, y=w323) -> (x != y?=w322:bool)
              n99 = call-dynamic "Skip all.vi"("error in (no error)"=w318, "Monkey in"=w319) -> ("error out"=w321:errorcluster, "Monkey out"=w320:refnum<class "Monkey.lvclass">)  [unwired: 8 in]
              n100 = case "#schedule-end" shown="True" w322 {
                tunnel: w321 -> [w326 w340]
                tunnel: [w328 w331] -> w317
                tunnel: [w327 w332] -> w316
                tunnel: w320 -> [w329 w339]
                tunnel: [w325 w333] -> w315
                tunnel: ["" w336] -> w314
                frame False {
                  # "This Monkey has nothing more in the scheule. Its job is done"
                  n101 = call-dynamic "All RUNs Completed.vi"("error in (no error)"=w326, "Monkey in"=w329) -> ("error out"=w327:errorcluster, "Monkey Status"=w325:T8, "Monkey out"=w328:refnum<class "Monkey.lvclass">)  [unwired: 7 in]
                }
                frame True {
                  # "Skip all RUNs if this Monkey is not empty"
                  # "There was something in the schedule (it is synced)."
                  n102 = call <vilib>:"Space Constant.vi"() -> ("String"=w347:string)
                  n103 = Concatenate Strings("Skip all scripts:" ("GUI Item Name"), w347, "synced with Kasli that finished!" ("string")) -> (w336:string)
                  n104 = call <vilib>:"Space Constant.vi"() -> ("String"=w344:string)
                  n105 = call "Update GUI.vi"("error in (no error)"=w340, "Data"=w336, "GUI Item Name"="Current Action", "uService Template in"=w339) -> ("error out"=w350:errorcluster, "uService Template out"=w351:refnum<class "Monkey.lvclass">)  [unwired: 6 in]
                  n106 = call "Date n Time.vi"() -> ("Date & Time"=w343:string)  [unwired: 5 in]
                  n107 = Concatenate Strings(w343, w344, w336) -> (w342:string)
                  n108 = call "Update GUI - Append String.vi"("Lines to keep"=u8 30, "error in (no error)"=w350, "String"=w342, "GUI Item Name"="Report from previous RUNs", "Father of all uServices in"=w351) -> ("error out"=w334:errorcluster, "Father of all uServices out"=w338:refnum<class "Monkey.lvclass">)  [unwired: 5 in]
                  n109 = Bundle By Name(cluster=w338, "STOPPED"=TRUE) -> (w335:refnum<class "Monkey.lvclass">)
                  n110 = call-dynamic "All RUNs Completed.vi"("error in (no error)"=w334, "Monkey in"=w335) -> ("error out"=w332:errorcluster, "Monkey Status"=w333:T8, "Monkey out"=w331:refnum<class "Monkey.lvclass">)  [unwired: 7 in]
                }
              }
            }
          }
          n111 = call-dynamic "Report to the Control uService.vi"("error in (no error)"=w195, "Current Action"=w192, "Monkey Status"=w193, "Monkey in"=w197) -> ("error out"=w194:errorcluster, "Monkey out"=w196:refnum<class "Monkey.lvclass">)  [unwired: 6 in]
        }
        frame "Quality Check" {
          # "To envoke the Quality Check, the Run had to return the All Good result. Check expected values in the DAQ. Retry the RUN if the condition is not met."
          n112 = Format Into String(format string="%s", error in=w354, w357) -> (resulting string=w356:string, error out=w353:errorcluster)  [unwired: 1 in]
          n113 = call "Update GUI.vi"("error in (no error)"=w353, "Data"=w356, "GUI Item Name"="Current Action", "uService Template in"=w365) -> ("error out"=w366:errorcluster, "uService Template out"=w358:refnum<class "Monkey.lvclass">)  [unwired: 6 in]
          n114 = Variant To Data(error in=w366, type=T10 {"FPGA Name"="", "Return Code"=enum."All Good"} ("Cluster"), Variant=w364) -> (data=w361:T10, error out=w360:errorcluster)
          n115 = case shown="No Error" w360 {
            selector: w360 -> [w384 w431]
            tunnel: [w369 w428] -> w363
            tunnel: [w368 w423] -> w352
            tunnel: w358 -> [w386 w424]
            tunnel: w361 -> [w381 _]
            frame No Error {
              n116 = Unbundle By Name(w381) -> ("Return Code"=w383:T11)
              n117 = call-dynamic "Max from Banana and Crit.vi"("error in (no error)"=w384, "Return Code"=w383, "Monkey in"=w386) -> ("error out"=w371:errorcluster, "Return Code"=w382:T11, "Monkey out"=w385:refnum<class "Monkey.lvclass">)  [unwired: 6 in]
              n118 = case shown="\"All Good\"" w382 {
                selector: w382 -> [w400 _]
                tunnel: w385 -> [w401 w406]
                tunnel: [w401 w403] -> w378
                tunnel: [w400 w405] -> w370
                tunnel: [_ w402] -> w367
                frame Default {
                  # "The overall result is higher than 0"
                }
                frame "All Good" {
                  # "The evaluation is OK, check the quality"
                  n119 = call-dynamic "Quality of Run Check.vi"("Monkey in"=w406) -> ("error out"=w404:errorcluster, "Check Result"=w405:T11, "Monkey out"=w403:refnum<class "Monkey.lvclass">)  [unwired: 8 in]
                  n120 = case shown="No Error" w404 {
                    selector: w404 -> [w409 w417]
                    tunnel: w405 -> [w415 _]
                    tunnel: w403 -> [w413 w418]
                    tunnel: [w408 w416] -> w402
                    frame No Error {
                      w407 = 5722  # #5722
                      n121 = call "Generate Error.vi"("Class"=w413, "Error Code"=w407) -> ("error out"=w410:errorcluster)  [unwired: 5 in]
                      n122 = Equal?(x=w415, y=Return_Code."All Good" ("x")) -> (x = y?=w412:bool)
                      n123 = Not(x=w412) -> (.not. x?=w411:bool)
                      n124 = Select(t=w410, s=w411, f=w409) -> (s? t:f=w408:errorcluster)
                    }
                    frame Error {
                      # "#5715"
                      n125 = call "Substitute Error.vi"("LabVIEW Object"=w418, "error in (no error)"=w417, "Error Code"=5715) -> ("error out"=w416:errorcluster)  [unwired: 8 in]
                    }
                  }
                }
              }
              n126 = call-dynamic "Check Optimisation Status.vi"("error in (no error)"=w371, "Monkey in"=w378) -> ("error out"=w376:errorcluster, "Optimiser"=w373:bool, "Monkey out"=w377:refnum<class "Monkey.lvclass">)  [unwired: 7 in]
              n127 = Bundle By Name(cluster=w381, "Return Code"=w370) -> (w380:T10)
              n128 = Equal?(x=Return_Code."All Good", y=w370) -> (x = y?=w374:bool)
              n129 = And(x=w373, y=w374) -> (x .and. y?=w372:bool)
              n130 = case shown="False" w372 {
                tunnel: w377 -> [w390 w399]
                tunnel: w376 -> [w392 w398]
                tunnel: [w391 w394] -> w369
                tunnel: [w387 w393] -> w379
                tunnel: w380 -> [w388 w395]
                frame True {
                  n131 = call "Send to Consumer.vi"("error in (no error)"=w392, "Data"=w388, "Case ID"=Monkey_Consumer_Case_Selector."Optimiser - evaluate RUN" ("Consumer Case Selector"), "uService Template in"=w390) -> ("error out"=w387:errorcluster, "uService Template out"=w391:refnum<class "Monkey.lvclass">)  [unwired: 6 in]
                }
                frame False {
                  n132 = global read "Global Constants.vi" "\"Smart\" uService"() -> (w396:string)
                  n133 = call "Message to uService.vi"("Father of all uServices in"=w399, "uService ID"=w396, "Message"="Quality Check - result", "Data"=w395, "error in (no error)"=w398) -> ("Father of all uServices out"=w394:refnum<class "Monkey.lvclass">, "error out"=w393:errorcluster)  [unwired: 9 in]
                }
              }
              n134 = Merge Errors(w367, w379) -> (w368:errorcluster)
            }
            frame Error {
              # "#5207"
              n135 = call "Substitute Error.vi"("LabVIEW Object"=w424, "error in (no error)"=w431, "Error Code"=5207, "Optional String"="Wrong format of the Banana in Quality Check!") -> ("error out"=w420:errorcluster)  [unwired: 7 in]
              n136 = global read "Global Constants.vi" "\"Smart\" uService"() -> (w422:string)
              n137 = property class="Monkey.lvclass"(reference=w424) -> (reference out=w427:refnum<class "Monkey.lvclass">, "Accessors:ID"=w426:string)  [unwired: 1 in, 1 out]
              n138 = call "Message to uService.vi"("Father of all uServices in"=w427, "uService ID"=w422, "Message"=" Quality Check - result", "Data"=w426) -> ("Father of all uServices out"=w428:refnum<class "Monkey.lvclass">, "error out"=w421:errorcluster)  [unwired: 10 in]
              n139 = Merge Errors(w420, w421) -> (w423:errorcluster)
            }
          }
        }
        frame "Optimiser - evaluate RUN" {
          n140 = call "Update GUI.vi"("error in (no error)"=w447, "Data"="Optimiser" ("GUI Item Name"), "GUI Item Name"="Current Action", "uService Template in"=w446) -> ("error out"=w433:errorcluster, "uService Template out"=w434:refnum<class "Monkey.lvclass">)  [unwired: 6 in]
          n141 = property class="Monkey.lvclass"(reference=w434, error in=w433) -> (reference out=w438:refnum<class "Monkey.lvclass">, error out=w439:errorcluster, "Accessors:Run Block"=w435:refnum<class "Run Block.lvclass">, "Accessors:Analysis Framework"=w432:refnum<class "Analysis Framework.lvclass">)
          n142 = call-dynamic "Get Optimiser Cell.vi"("error in (no error)"=w439, "Run Block in"=w435) -> ("error out"=w442:errorcluster, "Optimiser Cell"=w436:refnum<class "Optimiser Cell.lvclass">, "Run Block out"=w437:refnum<class "Run Block.lvclass">)  [unwired: 7 in]
          n143 = case shown="No Error" w442 {
            selector: w442 -> [w460 w521]
            tunnel: w438 -> [w468 w525]
            tunnel: w437 -> [w467 _]
            tunnel: w436 -> [w466 _]
            tunnel: w432 -> [w461 _]
            tunnel: [w453 w524] -> w444
            tunnel: w443 -> [w450 w523]
            tunnel: [w458 w522] -> w445
            frame No Error {
              # "#5713"
              n144 = call-dynamic "Calculate Observables.vi"("Analysis Framework"=w461, "error in (no error)"=w460, "Optimiser Cell in"=w466) -> ("error out"=w465:errorcluster, "Retry?"=w463:bool, "Optimiser Cell out"=w464:refnum<class "Optimiser Cell.lvclass">)  [unwired: 6 in]
              n145 = case shown="No Error" w465 {
                selector: w465 -> [w495 w519]
                tunnel: w464 -> [w497 w518]
                tunnel: w463 -> [w498 _]
                tunnel: [w496 w518] -> w462
                tunnel: [w493 _] -> w452
                tunnel: [w492 w517] -> w451
                tunnel: [w494 w519] -> w456
                tunnel: w450 -> [w491 w517]
                tunnel: [w490 _] -> w448
                frame No Error {
                  n146 = case shown="True" w498 {
                    tunnel: w497 -> [w503 w515]
                    tunnel: [w500 w515] -> w496
                    tunnel: w495 -> [w502 w508]
                    tunnel: [w501 w516] -> w494
                    tunnel: [Monkey_Consumer_Case_Selector."Optimiser - update RUN" ("Monkey Consumer Case Selector") Monkey_Consumer_Case_Selector."Optimiser - evaluate RUN" ("Monkey Consumer Case Selector")] -> w493
                    tunnel: [w499 w514] -> w492
                    tunnel: w491 -> [w499 w514]
                    tunnel: [_ w512] -> w490
                    frame False {
                      # "Observables calculated properly, ask optimiser for new set of parameters"
                      n147 = call-dynamic "Reset NaN Retries Counter.vi"("error in (no error)"=w502, "Run Optimiser in"=w503) -> ("error out"=w501:errorcluster, "Run Optimiser out"=w500:refnum<class "Optimiser Cell.lvclass">)  [unwired: 8 in]
                    }
                    frame True {
                      w509 = 5716  # #5716
                      # "NaN encountered, try reading the observable again"
                      n148 = call "TALOS Config Param.vi"("error in (no error)"=w508, "Parameter Name"="Optimiser_Wait_s") -> ("error out"=w507:errorcluster, "Output"=w505:string)  [unwired: 8 in]
                      n149 = Scan From String(input string=w505, error in=w507, default 1=5.0 ("default value 1")) -> (error out=w511:errorcluster, output 1=w512:dbl)  [unwired: 2 in, 2 out]
                      n150 = call "Substitute Error.vi"("LabVIEW Object"=w515, "error in (no error)"=w511, "Error Code"=w509) -> ("error out"=w516:errorcluster)  [unwired: 8 in]
                    }
                  }
                }
                frame Error {
                }
              }
              n151 = call-dynamic "Replace Scheduled Cell.vi"("Schedule Cell"=w462, "Run Block in"=w467) -> ("error out"=w457:errorcluster, "Run Block out"=w469:refnum<class "Run Block.lvclass">)  [unwired: 8 in]
              n152 = property class="Monkey.lvclass"(reference=w468, "Accessors:Run Block"=w469) -> (reference out=w454:refnum<class "Monkey.lvclass">)  [unwired: 1 in, 1 out]
              n153 = Merge Errors(w457, w456) -> (w455:errorcluster)
              n154 = case shown="No Error" w455 {
                selector: w455 -> [w474 w479]
                tunnel: w454 -> [w476 w489]
                tunnel: [w475 w486] -> w453
                tunnel: w452 -> [w473 _]
                tunnel: w451 -> [w472 w481]
                tunnel: [w471 w478] -> w449
                tunnel: w448 -> [w470 _]
                frame No Error {
                  n155 = call "Delayed Send to Consumer.vi"("Seconds (5)"=w470, "error in (no error)"=w474, "Data"=w472, "Case ID"=w473, "Father of all uServices in"=w476) -> ("error out"=w471:errorcluster, "Father of all uServices out"=w475:refnum<class "Monkey.lvclass">)  [unwired: 5 in]
                }
                frame Error {
                  # "If there was an error we want to skip this because something is wrong with the optimiser"
                  n156 = Variant To Data(type=T10 {"FPGA Name"="", "Return Code"=enum."All Good"} ("Cluster"), Variant=w481) -> (data=w484:T10, error out=w477:errorcluster)  [unwired: 1 in]
                  n157 = global read "Global Constants.vi" "\"Smart\" uService"() -> (w488:string)
                  n158 = Bundle By Name(cluster=w484, "Return Code"=Return_Code."Skip") -> (w483:T10)
                  n159 = call "Message to uService.vi"("Father of all uServices in"=w489, "uService ID"=w488, "Message"="Quality Check - result", "Data"=w483) -> ("Father of all uServices out"=w486:refnum<class "Monkey.lvclass">, "error out"=w480:errorcluster)  [unwired: 10 in]
                  n160 = Merge Errors(w480, w479, w477) -> (w478:errorcluster)
                }
              }
              n161 = call "Substitute Error.vi"("LabVIEW Object"=w453, "error in (no error)"=w449, "Error Code"=5713) -> ("error out"=w458:errorcluster)  [unwired: 8 in]
            }
            frame Error {
              # "Not the optimiser cell, so we can ignore it"
              n162 = call <vilib>:"Clear Errors.vi"("error in (no error)"=w521) -> ("error out"=w520:errorcluster)  [unwired: 5 in, 1 out]
              n163 = global read "Global Constants.vi" "\"Smart\" uService"() -> (w526:string)
              n164 = call "Message to uService.vi"("Father of all uServices in"=w525, "uService ID"=w526, "Message"="Quality Check - result", "Data"=w523, "error in (no error)"=w520) -> ("Father of all uServices out"=w524:refnum<class "Monkey.lvclass">, "error out"=w522:errorcluster)  [unwired: 9 in]
            }
          }
        }
        frame "Optimiser - update RUN" {
          # "Optimiser finished?\nIf it is finished -> remove the schedule cell from the schedule, go to the script checker.\nIf it isn't finished -> Get the new parameters, update the Schedule Cell (with new parameters in the Run Instance), go to the script checker"
          n165 = property class="Monkey.lvclass"(reference=w538) -> (reference out=w533:refnum<class "Monkey.lvclass">, "Accessors:Analysis Framework"=w528:refnum<class "Analysis Framework.lvclass">, "Accessors:Run Block"=w529:refnum<class "Run Block.lvclass">)  [unwired: 1 in, 1 out]
          n166 = call-dynamic "Get Optimiser Cell.vi"("error in (no error)"=w537, "Run Block in"=w529) -> ("error out"=w530:errorcluster, "Optimiser Cell"=w531:refnum<class "Optimiser Cell.lvclass">, "Run Block out"=w532:refnum<class "Run Block.lvclass">)  [unwired: 7 in]
          n167 = case shown="No Error" w530 {
            selector: w530 -> [w555 w609]
            tunnel: w533 -> [w562 w606]
            tunnel: w532 -> [w561 _]
            tunnel: [w540 w604] -> w536
            tunnel: w531 -> [w556 _]
            tunnel: w528 -> [w551 _]
            tunnel: [w547 w605] -> w535
            tunnel: w534 -> [w543 w600]
            frame No Error {
              # "#5714"
              n168 = call-dynamic "Run Optimiser.vi"("Analysis Framework"=w551, "error in (no error)"=w555, "Optimiser Cell in"=w556) -> ("error out"=w552:errorcluster, "Optimiser Cell out"=w553:refnum<class "Optimiser Cell.lvclass">, "Optimiser Finished"=w554:bool)  [unwired: 6 in]
              n169 = call-dynamic "Replace Scheduled Cell.vi"("error in (no error)"=w552, "Schedule Cell"=w553, "Run Block in"=w561) -> ("error out"=w557:errorcluster, "Run Block out"=w560:refnum<class "Run Block.lvclass">)  [unwired: 7 in]
              n170 = property class="Monkey.lvclass"(reference=w562, "Accessors:Run Block"=w560) -> (reference out=w558:refnum<class "Monkey.lvclass">)  [unwired: 1 in, 1 out]
              n171 = case shown="True" w554 {
                tunnel: w558 -> [w567 w586]
                tunnel: [w566 w585] -> w548
                tunnel: w557 -> [w569 w584]
                tunnel: [w568 w593] -> w545
                tunnel: w543 -> [w565 w583]
                tunnel: [w563 w583] -> w539
                tunnel: [errorcluster {"status"=FALSE, "code"=0, "source"=""} ("error out") w581] -> w541
                frame False {
                  # "Optimisation not reached"
                  n172 = case shown="No Error" w569 {
                    selector: w569 -> [w571 w575]
                    tunnel: [w571 w580] -> w568
                    tunnel: w567 -> [w572 w579]
                    tunnel: [w572 w579] -> w566
                    tunnel: w565 -> [w570 w574]
                    tunnel: [w570 w577] -> w563
                    frame No Error {
                    }
                    frame Error {
                      n173 = Variant To Data(error in=w575, type=T10 {"FPGA Name"="", "Return Code"=enum."All Good"} ("Cluster"), Variant=w574) -> (data=w573:T10, error out=w580:errorcluster)
                      n174 = Bundle By Name(cluster=w573, "Return Code"=Return_Code."Skip") -> (w577:T10)
                    }
                  }
                }
                frame True {
                  # "Optimisation reached"
                  n175 = call-dynamic "Run Best Optimisation Parameters.vi"("error in (no error)"=w584, "Monkey in"=w586) -> ("error out"=w593:errorcluster, "Best Parameters"=w582:string[][], "Monkey out"=w585:refnum<class "Monkey.lvclass">)  [unwired: 7 in]
                  n176 = for {
                    tunnel: w582 -> [w596] mode=indexing
                    tunnel: [w594] -> w590 mode=indexing
                    n177 = call <vilib>:"1D String Array to Delimited String.vi"("delimiter"="=", "string array"=w596) -> ("delimited string"=w594:string)  [unwired: 9 in]
                  }
                  n178 = call <vilib>:"1D String Array to Delimited String.vi"("delimiter"="\r", "string array"=w590) -> ("delimited string"=w588:string)  [unwired: 9 in]
                  n179 = Concatenate Strings("Optimiser finished. Best parameters are:\n" ("Text"), w588) -> (w587:string)
                  n180 = call "Temporised Pop-up Window.vi"("Timeout"=5.0, "Text"=w587) -> ("error out"=w581:errorcluster)  [unwired: 9 in]
                }
              }
              n181 = global read "Global Constants.vi" "\"Smart\" uService"() -> (w550:string)
              n182 = call "Message to uService.vi"("Father of all uServices in"=w548, "uService ID"=w550, "Message"="Quality Check - result", "Data"=w539) -> ("Father of all uServices out"=w547:refnum<class "Monkey.lvclass">, "error out"=w546:errorcluster)  [unwired: 10 in]
              n183 = Merge Errors(w546, w545) -> (w544:errorcluster)
              n184 = call "Substitute Error.vi"("LabVIEW Object"=w547, "error in (no error)"=w544, "Error Code"=5714) -> ("error out"=w542:errorcluster)  [unwired: 8 in]
              n185 = Merge Errors(w542, w541) -> (w540:errorcluster)
            }
            frame Error {
              # "Just in case, let the Tamer know that something is up"
              # "Not an optimise cell, this should be impossible to reach"
              n186 = Variant To Data(type=T10 {"FPGA Name"="", "Return Code"=enum."All Good"} ("Cluster"), Variant=w600) -> (data=w601:T10, error out=w597:errorcluster)  [unwired: 1 in]
              n187 = global read "Global Constants.vi" "\"Smart\" uService"() -> (w607:string)
              n188 = Bundle By Name(cluster=w601, "Return Code"=Return_Code."Skip") -> (w599:T10)
              n189 = call "Message to uService.vi"("Father of all uServices in"=w606, "uService ID"=w607, "Message"=" Quality Check - result", "Data"=w599) -> ("Father of all uServices out"=w605:refnum<class "Monkey.lvclass">, "error out"=w598:errorcluster)  [unwired: 10 in]
              n190 = Merge Errors(w598, w597, w609) -> (w604:errorcluster)
            }
          }
        }
        frame "Banana arrived" {
          # "This case is needed to avoid the race condition of an error getting enqueued immediately after the Run is finished: the Monkey would then skip the Criticality Level associated to that error (and, by the way, using it in the subsequent Run). In this way, the \"What to do next\" will be enqued after any - reasonably - possible \"Error Criticality\" message from the Error Manager."
          n191 = call "Send to Consumer.vi"("error in (no error)"=w612, "Data"=w611, "Case ID"=Monkey_Consumer_Case_Selector."What to do next" ("Consumer Case Selector"), "uService Template in"=w613) -> ("error out"=w614:errorcluster, "uService Template out"=w616:refnum<class "Monkey.lvclass">)  [unwired: 6 in]
          n192 = in-place {
            # "Calculate average time per script"
            n193 = in-place-cluster #1(w616) -> ("Last run start"=w622:timestamp, "Times of last N runs"=w625:dbl[], "N"=w620:u32)  [unwired: 1 out]
            n194 = Get Date/Time In Seconds() -> (seconds since 1Jan1904=w626:timestamp)
            n195 = Subtract(x=w626, y=w622) -> (x-y=w624:dbl)
            n196 = Insert Into Array(array=w625, new element=w624) -> (w623:dbl[])  [unwired: 1 in]
            n197 = Array Size(array=w623) -> (size(s)=w628:i32)
            n198 = Greater?(x=w628, y=w620) -> (0:w627:bool)
            n199 = case shown="True" w627 {
              tunnel: w623 -> [w629 w632]
              tunnel: [w629 w630] -> w618
              frame False {
              }
              frame True {
                # "This will be 11th point, remove the first one (oldest)"
                n200 = Delete From Array(array=w632, index=0) -> (array with subset deleted=w630:dbl[])  [unwired: 1 in, 1 out]
              }
            }
            n201 = Array Size(array=w618) -> (size(s)=w617:i32)
            n202 = Add Array Elements(numeric array=w618) -> (sum=w621:dbl)
            n203 = Divide(x=w621, y=w617) -> (x/y=w619:dbl)
            n204 = in-place-cluster #1("Last run start"=w622, "Times of last N runs"=w618, "Average time per script"=w619, "N"=w620) -> (w615:refnum<class "Monkey.lvclass">)
          }
        }
        frame "What to do next" {
          n205 = Variant To Data(error in=w645, type=u16 0, Variant=w646) -> (data=w639:u16, error out=w640:errorcluster)
          n206 = case shown="Error .." w640 {
            selector: w640 -> [w851 w856]
            tunnel: w639 -> [w852 _]
            tunnel: [w852 u16 3] -> w634
            tunnel: [w851 w855] -> w633
            tunnel: w642 -> [_ w853]
            frame No Error {
            }
            frame Error {
              # "#5703"
              n207 = call "Substitute Error.vi"("LabVIEW Object"=w853, "error in (no error)"=w856, "Error Code"=5703) -> ("error out"=w855:errorcluster)  [unwired: 8 in]
            }
          }
          n208 = case shown="4" w634 {
            selector: w634 -> [_ w708 w750 w814 w845]
            tunnel: w633 -> [w654 w710 w752 w808 w838]
            tunnel: w642 -> [w653 w709 w751 w810 w839]
            tunnel: [w658 w705 w744 w806 w840] -> w638
            tunnel: [w659 w704 w743 w805 w837] -> w635
            tunnel: w634 -> [_ _ _ w813 _]
            tunnel: [w655 w698 w746 w802 Monkey_Status."Finished (with errors)" ("Monkey Status")] -> w637
            frame 0 {
              # "All good! Go to the next RUN on the list."
              n209 = call "Update Report Previous RUNs.vi"("error in (no error)"=w654, "Previous RUN outcome"=" finished well!" ("string"), "Monkey in"=w653) -> ("error out"=w650:errorcluster, "Monkey out"=w651:refnum<class "Monkey.lvclass">)  [unwired: 7 in]
              n210 = call-dynamic "The End of the RUN.vi"("error in (no error)"=w650, "Monkey in"=w651) -> ("error out"=w648:errorcluster, "Monkey out"=w649:refnum<class "Monkey.lvclass">)  [unwired: 8 in]
              n211 = call-dynamic "Get Schedule Status.vi"("error in (no error)"=w648, "Monkey in"=w649) -> ("error out"=w652:errorcluster, "Empty?"=w656:bool, "Monkey out"=w657:refnum<class "Monkey.lvclass">)  [unwired: 6 in, 1 out]
              n212 = case shown="True" w656 {
                tunnel: [w668 w682] -> w659
                tunnel: [w667 w683] -> w658
                tunnel: w657 -> [w671 w679]
                tunnel: w652 -> [w662 w680]
                tunnel: [Monkey_Status."Ongoing" ("Monkey Status") w681] -> w655
                frame False {
                  # "More scripts to go"
                  n213 = call "Send to Consumer.vi"("error in (no error)"=w662, "Case ID"=Monkey_Consumer_Case_Selector."Update GUI" ("Consumer Case Selector"), "uService Template in"=w671) -> ("error out"=w660:errorcluster, "uService Template out"=w672:refnum<class "Monkey.lvclass">)  [unwired: 7 in]
                  n214 = call "Send to Consumer.vi"("error in (no error)"=w660, "Case ID"=Monkey_Consumer_Case_Selector."Check Script" ("Consumer Case Selector"), "uService Template in"=w672) -> ("error out"=w670:errorcluster, "uService Template out"=w669:refnum<class "Monkey.lvclass">)  [unwired: 7 in]
                  n215 = call "Update GUI.vi"("error in (no error)"=w670, "Data"="Next RUN!" ("GUI Item Name"), "GUI Item Name"="Current Action", "uService Template in"=w669) -> ("error out"=w668:errorcluster, "uService Template out"=w667:refnum<class "Monkey.lvclass">)  [unwired: 6 in]
                }
                frame True {
                  # "List's empty, means we've finished!"
                  n216 = call "Get GUI Item Value - Bool.vi"("error in (no error)"=w680, "FP Item Name"="Synchronised", "uService Template in"=w679) -> ("error out"=w676:errorcluster, "Value"=w673:bool, "uService Template out"=w677:refnum<class "Monkey.lvclass">)  [unwired: 6 in]
                  n217 = case shown="True" w673 {
                    tunnel: w677 -> [w685 w697]
                    tunnel: w676 -> [w684 w694]
                    tunnel: [w685 w689] -> w675
                    tunnel: [w684 w688] -> w674
                    frame False {
                      # "Stand-alone Monkey, no need to contact the Control uService"
                    }
                    frame True {
                      # "Synchronised process -> Contact the Control uService"
                      n218 = property class="Monkey.lvclass"(reference=w697, error in=w694) -> (reference out=w696:refnum<class "Monkey.lvclass">, error out=w695:errorcluster, "Accessors:ID"=w692:string)
                      n219 = Bundle By Name(cluster=T6 {"Monkey ID"="", "Script Checker Result"=enum."Passed"} ("Message"), "Monkey ID"=w692, "Script Checker Result"=Script_Checker_Result."Empty") -> (w691:T6)
                      n220 = global read "Global Constants.vi" "\"Smart\" uService"() -> (w686:string)
                      n221 = call "Message to uService.vi"("Father of all uServices in"=w696, "uService ID"=w686, "Message"="Script Checker", "Data"=w691, "error in (no error)"=w695) -> ("Father of all uServices out"=w689:refnum<class "Monkey.lvclass">, "error out"=w688:errorcluster)  [unwired: 9 in]
                    }
                  }
                  n222 = call-dynamic "All RUNs Completed.vi"("error in (no error)"=w674, "Monkey in"=w675) -> ("error out"=w682:errorcluster, "Monkey Status"=w681:T8, "Monkey out"=w683:refnum<class "Monkey.lvclass">)  [unwired: 7 in]
                }
              }
            }
            frame 1 {
              # "The RUN didn't go well: re-execute the script"
              n223 = Format Into String(format string=" %s %d. %s", error in=w710, "finished with error code:" ("initial string"), w708, "Retry another time" ("initial string")) -> (resulting string=w714:string, error out=w715:errorcluster)  [unwired: 1 in]
              n224 = call "Update Report Previous RUNs.vi"("error in (no error)"=w715, "Previous RUN outcome"=w714, "Monkey in"=w709) -> ("error out"=w699:errorcluster, "Monkey out"=w700:refnum<class "Monkey.lvclass">)  [unwired: 7 in]
              n225 = Unbundle By Name(w700) -> ("STOPPED"=w702:bool)
              n226 = case shown="False" w702 {
                tunnel: w700 -> [w721 w732]
                tunnel: [w728 w736] -> w706
                tunnel: [w727 w737] -> w703
                tunnel: w699 -> [w720 w731]
                tunnel: ["Next RUN!" ("GUI Item Name") "Runs stopped! Last script finished" ("Text to log")] -> w701
                tunnel: [Monkey_Status."Ongoing" ("Monkey Status") w733] -> w698
                frame False {
                  n227 = call-dynamic "Retry RUN.vi"("error in (no error)"=w720, "Next?"=TRUE, "Monkey in"=w721) -> ("error out"=w719:errorcluster, "Monkey out"=w717:refnum<class "Monkey.lvclass">)  [unwired: 7 in]
                  n228 = call "Send to Consumer.vi"("error in (no error)"=w719, "Case ID"=Monkey_Consumer_Case_Selector."Update GUI" ("Consumer Case Selector"), "uService Template in"=w717) -> ("error out"=w725:errorcluster, "uService Template out"=w716:refnum<class "Monkey.lvclass">)  [unwired: 7 in]
                  n229 = call "Send to Consumer.vi"("error in (no error)"=w725, "Case ID"=Monkey_Consumer_Case_Selector."Check Script" ("Consumer Case Selector"), "uService Template in"=w716) -> ("error out"=w728:errorcluster, "uService Template out"=w727:refnum<class "Monkey.lvclass">)  [unwired: 7 in]
                }
                frame True {
                  n230 = call-dynamic "Skip all.vi"("error in (no error)"=w731, "Monkey in"=w732) -> ("error out"=w729:errorcluster, "Monkey out"=w730:refnum<class "Monkey.lvclass">)  [unwired: 8 in]
                  n231 = call-dynamic "All RUNs Completed.vi"("error in (no error)"=w729, "Monkey in"=w730) -> ("error out"=w734:errorcluster, "Monkey Status"=w733:T8, "Monkey out"=w735:refnum<class "Monkey.lvclass">)  [unwired: 7 in]
                  n232 = call "Send to Consumer.vi"("error in (no error)"=w734, "Case ID"=Monkey_Consumer_Case_Selector."Update GUI" ("Consumer Case Selector"), "uService Template in"=w735) -> ("error out"=w736:errorcluster, "uService Template out"=w737:refnum<class "Monkey.lvclass">)  [unwired: 7 in]
                }
              }
              n233 = call "Update GUI.vi"("error in (no error)"=w706, "Data"=w701, "GUI Item Name"="Current Action", "uService Template in"=w703) -> ("error out"=w704:errorcluster, "uService Template out"=w705:refnum<class "Monkey.lvclass">)  [unwired: 6 in]
            }
            frame 2 {
              # "Skip the Run"
              n234 = Format Into String(format string=" %s %d. %s", error in=w752, "finished with error code:" ("initial string"), w750, "Skipping it and moving to the next one." ("initial string")) -> (resulting string=w756:string, error out=w757:errorcluster)  [unwired: 1 in]
              n235 = call "Update Report Previous RUNs.vi"("error in (no error)"=w757, "Previous RUN outcome"=w756, "Monkey in"=w751) -> ("error out"=w747:errorcluster, "Monkey out"=w748:refnum<class "Monkey.lvclass">)  [unwired: 7 in]
              n236 = Unbundle By Name(w748) -> ("STOPPED"=w749:bool)
              n237 = case shown="False" w749 {
                tunnel: w748 -> [w762 w788]
                tunnel: [w768 w793] -> w742
                tunnel: [w767 w794] -> w745
                tunnel: w747 -> [w759 w787]
                tunnel: [w766 "Runs stopped! Last script finished" ("Text to log")] -> w741
                tunnel: [w758 w790] -> w746
                frame False {
                  n238 = call-dynamic "Skip Current RUN.vi"("error in (no error)"=w759, "Monkey in"=w762) -> ("error out"=w760:errorcluster, "Monkey out"=w761:refnum<class "Monkey.lvclass">)  [unwired: 8 in]
                  n239 = call-dynamic "Get Schedule Status.vi"("error in (no error)"=w760, "Monkey in"=w761) -> ("error out"=w763:errorcluster, "Empty?"=w765:bool, "Monkey out"=w764:refnum<class "Monkey.lvclass">)  [unwired: 6 in, 1 out]
                  n240 = case shown="True" w765 {
                    tunnel: [w778 w781] -> w768
                    tunnel: [w777 w780] -> w767
                    tunnel: ["Next RUN!" ("GUI Item Name") "All the RUNs completed!" ("Text to log")] -> w766
                    tunnel: w764 -> [w772 w783]
                    tunnel: w763 -> [w775 w782]
                    tunnel: [Monkey_Status."Ongoing" ("Monkey Status") w779] -> w758
                    frame False {
                      # "More scripts to go"
                      n241 = call "Send to Consumer.vi"("error in (no error)"=w775, "Case ID"=Monkey_Consumer_Case_Selector."Update GUI" ("Consumer Case Selector"), "uService Template in"=w772) -> ("error out"=w774:errorcluster, "uService Template out"=w771:refnum<class "Monkey.lvclass">)  [unwired: 7 in]
                      n242 = call "Send to Consumer.vi"("error in (no error)"=w774, "Case ID"=Monkey_Consumer_Case_Selector."Check Script" ("Consumer Case Selector"), "uService Template in"=w771) -> ("error out"=w778:errorcluster, "uService Template out"=w777:refnum<class "Monkey.lvclass">)  [unwired: 7 in]
                    }
                    frame True {
                      # "Empty schedule"
                      n243 = call-dynamic "All RUNs Completed.vi"("error in (no error)"=w782, "Monkey in"=w783) -> ("error out"=w781:errorcluster, "Monkey Status"=w779:T8, "Monkey out"=w780:refnum<class "Monkey.lvclass">)  [unwired: 7 in]
                    }
                  }
                }
                frame True {
                  n244 = call-dynamic "Skip all.vi"("error in (no error)"=w787, "Monkey in"=w788) -> ("error out"=w785:errorcluster, "Monkey out"=w786:refnum<class "Monkey.lvclass">)  [unwired: 8 in]
                  n245 = call-dynamic "All RUNs Completed.vi"("error in (no error)"=w785, "Monkey in"=w786) -> ("error out"=w791:errorcluster, "Monkey Status"=w790:T8, "Monkey out"=w792:refnum<class "Monkey.lvclass">)  [unwired: 7 in]
                  n246 = call "Send to Consumer.vi"("error in (no error)"=w791, "Case ID"=Monkey_Consumer_Case_Selector."Update GUI" ("Consumer Case Selector"), "uService Template in"=w792) -> ("error out"=w793:errorcluster, "uService Template out"=w794:refnum<class "Monkey.lvclass">)  [unwired: 7 in]
                }
              }
              n247 = call "Update GUI.vi"("error in (no error)"=w742, "Data"=w741, "GUI Item Name"="Current Action", "uService Template in"=w745) -> ("error out"=w743:errorcluster, "uService Template out"=w744:refnum<class "Monkey.lvclass">)  [unwired: 6 in]
            }
            frame 3, Default {
              # "Recieved stop or Something went wrong, stop all the RUNs (and recheck the uServices??)"
              n248 = Unbundle By Name(w810) -> ("STOPPED"=w815:bool)
              n249 = case shown="False" w815 {
                tunnel: w814 -> [w825 _]
                tunnel: w813 -> [_ w829]
                tunnel: ["There was a crash!!!!" ("GUI Item Name") "Runs stopped!" ("Text to log")] -> w797
                tunnel: ["Skipping everything, clearing the queue" ("initial string") "STOPPED! Skipping everything, clearing the queue" ("initial string")] -> w812
                tunnel: [w825 w829] -> w811
                tunnel: w810 -> [w822 w828]
                tunnel: [w822 w828] -> w809
                tunnel: w808 -> [w821 w827]
                tunnel: [w821 w827] -> w807
                tunnel: [Monkey_Status."Finished (with errors)" ("Monkey Status") Monkey_Status."Stopped" ("Monkey Status")] -> w802
                frame False {
                  # "CRASH"
                }
                frame True {
                  # "STOP"
                }
              }
              n250 = Format Into String(format string=" %s %d. %s", error in=w807, "finished with error code:" ("initial string"), w811, w812) -> (resulting string=w818:string, error out=w819:errorcluster)  [unwired: 1 in]
              n251 = call "Update Report Previous RUNs.vi"("error in (no error)"=w819, "Previous RUN outcome"=w818, "Monkey in"=w809) -> ("error out"=w803:errorcluster, "Monkey out"=w804:refnum<class "Monkey.lvclass">)  [unwired: 7 in]
              n252 = call-dynamic "Skip all.vi"("error in (no error)"=w803, "Monkey in"=w804) -> ("error out"=w800:errorcluster, "Monkey out"=w801:refnum<class "Monkey.lvclass">)  [unwired: 8 in]
              n253 = call-dynamic "All RUNs Completed.vi"("error in (no error)"=w800, "Monkey in"=w801) -> ("error out"=w798:errorcluster, "Monkey out"=w799:refnum<class "Monkey.lvclass">)  [unwired: 7 in, 1 out]
              n254 = call "Update GUI.vi"("error in (no error)"=w798, "Data"=w797, "GUI Item Name"="Current Action", "uService Template in"=w799) -> ("error out"=w805:errorcluster, "uService Template out"=w806:refnum<class "Monkey.lvclass">)  [unwired: 6 in]
            }
            frame 4 {
              # "Something went horribly wrong, ABORT everything and run for your life"
              n255 = Format Into String(format string=" %s %d. %s", error in=w838, "finished with error code:" ("initial string"), w845, "Skipping everything!! ABORT!!" ("initial string")) -> (resulting string=w849:string, error out=w850:errorcluster)  [unwired: 1 in]
              n256 = call "Update Report Previous RUNs.vi"("error in (no error)"=w850, "Previous RUN outcome"=w849, "Monkey in"=w839) -> ("error out"=w841:errorcluster, "Monkey out"=w842:refnum<class "Monkey.lvclass">)  [unwired: 7 in]
              n257 = call-dynamic "Skip all.vi"("error in (no error)"=w841, "Monkey in"=w842) -> ("error out"=w832:errorcluster, "Monkey out"=w835:refnum<class "Monkey.lvclass">)  [unwired: 8 in]
              n258 = call-dynamic "All RUNs Completed.vi"("error in (no error)"=w832, "Monkey in"=w835) -> ("error out"=w833:errorcluster, "Monkey out"=w834:refnum<class "Monkey.lvclass">)  [unwired: 7 in, 1 out]
              n259 = call "Update GUI.vi"("error in (no error)"=w833, "Data"="Something went horribly wrong!!!!" ("GUI Item Name"), "GUI Item Name"="Current Action", "uService Template in"=w834) -> ("error out"=w837:errorcluster, "uService Template out"=w840:refnum<class "Monkey.lvclass">)  [unwired: 6 in]
            }
          }
          n260 = call-dynamic "Report to the Control uService.vi"("Monkey Status"=w637, "Monkey in"=w638) -> ("error out"=w636:errorcluster, "Monkey out"=w644:refnum<class "Monkey.lvclass">)  [unwired: 8 in]
          n261 = Merge Errors(w636, w635) -> (w643:errorcluster)
        }
        frame "Update Crit Lvl" {
          # "Should it be 3 or 0?\nIf someone forgets to put error criticality in the file, then we can assume it is 0. It is safer to keep as 3 though"
          # "If there was an error in variant to data, it means that the variant was empty: no specific error was provided. Ignore that error"
          # "Stop or ABORT?\nThis is handled by Tamer now. Monkey only deals with 0,1,2"
          n262 = global read "Global Constants.vi" "ABORT Crt Lvl"() -> (w862:u8)
          n263 = Variant To Data(error in=w874, type=u8 0, Variant=w875) -> (data=w867:u8, error out=w868:errorcluster)
          n264 = case shown="Error .." w868 {
            selector: w868 -> [w885 w890]
            tunnel: w867 -> [w886 _]
            tunnel: [w886 w887] -> w866
            tunnel: [w885 w889] -> w865
            tunnel: w862 -> [_ w888]
            frame No Error {
            }
            frame Error {
              n265 = call <vilib>:"Clear Errors.vi"("error in (no error)"=w890) -> ("error out"=w889:errorcluster)  [unwired: 5 in, 1 out]
              n266 = Decrement(x=w888) -> (x-1=w887:u8)
            }
          }
          n267 = In Range and Coerce(upper limit=w862, x=w866, lower limit=u8 0) -> (In Range?=w858:bool)  [unwired: 1 out]
          n268 = case shown="True" w858 {
            tunnel: w866 -> [_ w881]
            tunnel: w865 -> [_ w880]
            tunnel: [w879 w880] -> w871
            tunnel: [w877 w881] -> w873
            tunnel: w862 -> [w877 _]
            tunnel: w860 -> [w876 _]
            frame False {
              # "#5702"
              n269 = call "Generate Error.vi"("Class"=w876, "Error Code"=5702) -> ("error out"=w879:errorcluster)  [unwired: 5 in]
            }
            frame True {
              # "All good!"
            }
          }
          n270 = in-place {
            in-place-border: w873 -> [w882]
            in-place-border: [w884] -> w864
            n271 = in-place-cluster #2(w860) -> ("Criticality Level"=w883:u8)
            n272 = Max & Min(x=w883, y=w882) -> (max(x,y)=w884:u8)  [unwired: 1 out]
            n273 = in-place-cluster #2("Criticality Level"=w884) -> (w872:refnum<class "Monkey.lvclass">)
          }
          n274 = call "Update GUI.vi"("error in (no error)"=w871, "Data"=w864, "GUI Item Name"="Error Criticality", "uService Template in"=w872) -> ("error out"=w869:errorcluster, "uService Template out"=w870:refnum<class "Monkey.lvclass">)  [unwired: 6 in]
        }
        frame "Skip Run" {
          w901 = FALSE
          n275 = property class="Monkey.lvclass"(reference=w895) -> (reference out=w894:refnum<class "Monkey.lvclass">, "Accessors:STOPPED"=w892:bool)  [unwired: 1 in, 1 out]
          n276 = Variant To Data(type=w901, Variant=w899) -> (data=w902:bool, error out=w903:errorcluster)  [unwired: 1 in]
          n277 = Select(t=w901, s=w903, f=w902) -> (s? t:f=w900:bool)
          n278 = call-dynamic "Get FPGA uService ID.vi"("Monkey in"=w894) -> ("FPGA uService ID"=w896:string, "Monkey out"=w904:refnum<class "Monkey.lvclass">)  [unwired: 8 in, 1 out]
          n279 = Empty String/Path?(string/path=w896) -> (empty?=w893:bool)
          n280 = Or(x=w893, y=w892) -> (x .or. y?=w891:bool)
          n281 = case shown="False" w891 {
            tunnel: w905 -> [w919 w933]
            tunnel: w904 -> [w918 w934]
            tunnel: w896 -> [w906 _]
            tunnel: w900 -> [w917 _]
            tunnel: [w913 w934] -> w898
            tunnel: [w912 w933] -> w897
            frame False {
              n282 = call "Message to uService.vi"("Father of all uServices in"=w918, "uService ID"=w906, "Message"="Terminate Script", "Data"=w917, "error in (no error)"=w919) -> ("Father of all uServices out"=w916:refnum<class "Monkey.lvclass">, "error out"=w915:errorcluster)  [unwired: 9 in]
              n283 = case shown="False" w917 {
                tunnel: w916 -> [w927 w932]
                tunnel: w915 -> [w925 w931]
                tunnel: [w923 w932] -> w914
                tunnel: [w922 w931] -> w911
                tunnel: ["" w928] -> w909
                frame False {
                  # "Not gracefully, means we need to finish this Run manually"
                  n284 = call "Send to Consumer.vi"("error in (no error)"=w925, "Data"=u16 2, "Case ID"=Monkey_Consumer_Case_Selector."What to do next" ("Monkey Consumer Case Selector"), "uService Template in"=w927) -> ("error out"=w922:errorcluster, "uService Template out"=w923:refnum<class "Monkey.lvclass">)  [unwired: 6 in]
                }
                frame True {
                  # "Gracefully, the script's closure function will be executed and the"
                  n285 = call <vilib>:"Space Constant.vi"() -> ("String"=w929:string)
                  n286 = Concatenate Strings(w929, "(with grace)" ("GUI Item Name")) -> (w928:string)
                }
              }
              n287 = Concatenate Strings("Skipping script" ("string"), w909) -> (w908:string)
              n288 = call "Update GUI.vi"("error in (no error)"=w911, "Data"=w908, "GUI Item Name"="Current Action", "uService Template in"=w914) -> ("error out"=w912:errorcluster, "uService Template out"=w913:refnum<class "Monkey.lvclass">)  [unwired: 6 in]
            }
            frame True {
              # "Nothing to skip or stpped already"
            }
          }
        }
        frame "Stop Schedule" {
          w939 = T16 {"Old value"=FALSE, "Gracefully?"=FALSE} ("Stop msg")
          n289 = Variant To Data(type=w939, Variant=w945) -> (data=w948:T16, error out=w949:errorcluster)  [unwired: 1 in]
          n290 = Select(t=w939, s=w949, f=w948) -> (s? t:f=w938:T16)
          n291 = Unbundle By Name(w938) -> ("Old value"=w937:bool, "Gracefully?"=w936:bool)
          n292 = call-dynamic "Get FPGA uService ID.vi"("Monkey in"=w935) -> ("FPGA uService ID"=w941:string, "Monkey out"=w946:refnum<class "Monkey.lvclass">)  [unwired: 8 in, 1 out]
          n293 = Empty String/Path?(string/path=w941) -> (empty?=w940:bool)
          n294 = Or(x=w940, y=w937) -> (x .or. y?=w942:bool)
          n295 = case shown="False" w942 {
            tunnel: w947 -> [w963 w977]
            tunnel: w946 -> [w961 w978]
            tunnel: w941 -> [w960 _]
            tunnel: w936 -> [w959 _]
            tunnel: [w955 w978] -> w944
            tunnel: [w954 w977] -> w943
            frame False {
              n296 = call "Message to uService.vi"("Father of all uServices in"=w961, "uService ID"=w960, "Message"="Terminate Script", "Data"=w959, "error in (no error)"=w963) -> ("Father of all uServices out"=w958:refnum<class "Monkey.lvclass">, "error out"=w957:errorcluster)  [unwired: 9 in]
              n297 = case shown="False" w959 {
                tunnel: w958 -> [w971 w976]
                tunnel: w957 -> [w969 w975]
                tunnel: [w967 w976] -> w956
                tunnel: [w966 w975] -> w953
                tunnel: ["" w972] -> w951
                frame False {
                  # "Not gracefully, means we need to finish this Run manually"
                  n298 = call "Send to Consumer.vi"("error in (no error)"=w969, "Data"=u16 3, "Case ID"=Monkey_Consumer_Case_Selector."What to do next" ("Monkey Consumer Case Selector"), "uService Template in"=w971) -> ("error out"=w966:errorcluster, "uService Template out"=w967:refnum<class "Monkey.lvclass">)  [unwired: 6 in]
                }
                frame True {
                  # "Gracefully, the script's closure function will be executed and the"
                  n299 = call <vilib>:"Space Constant.vi"() -> ("String"=w973:string)
                  n300 = Concatenate Strings(w973, "(with grace)" ("GUI Item Name")) -> (w972:string)
                }
              }
              n301 = Concatenate Strings("Stoppig Schedule" ("string"), w951) -> (w950:string)
              n302 = call "Update GUI.vi"("error in (no error)"=w953, "Data"=w950, "GUI Item Name"="Current Action", "uService Template in"=w956) -> ("error out"=w954:errorcluster, "uService Template out"=w955:refnum<class "Monkey.lvclass">)  [unwired: 6 in]
            }
            frame True {
              # "Nothing to stop"
            }
          }
        }
        frame "Skip schedule" {
          n303 = call-dynamic "Skip schedule.vi"("error in (no error)"=w988, "Monkey in"=w989) -> ("error out"=w986:errorcluster, "Monkey out"=w987:refnum<class "Monkey.lvclass">)  [unwired: 8 in]
          n304 = call "Update GUI.vi"("error in (no error)"=w986, "Data"=FALSE, "GUI Item Name"="Skip schedule", "uService Template in"=w987) -> ("error out"=w982:errorcluster, "uService Template out"=w981:refnum<class "Monkey.lvclass">)  [unwired: 6 in]
          n305 = call "Send to Consumer.vi"("error in (no error)"=w982, "Case ID"=Monkey_Consumer_Case_Selector."Update GUI" ("Monkey Consumer Case Selector"), "uService Template in"=w981) -> ("error out"=w980:errorcluster, "uService Template out"=w979:refnum<class "Monkey.lvclass">)  [unwired: 7 in]
        }
        frame "Update index" {
          w999 = -1
          n306 = Variant To Data(type=w999, Variant=w1001) -> (data=w998:i32, error out=w1000:errorcluster)  [unwired: 1 in]
          n307 = Select(t=w999, s=w1000, f=w998) -> (s? t:f=w993:i32)
          n308 = call-dynamic "Update Index Selector.vi"("error in (no error)"=w991, "Index selector"=w993, "Monkey in"=w994) -> ("error out"=w990:errorcluster, "Monkey out"=w992:refnum<class "Monkey.lvclass">)  [unwired: 7 in]
          n309 = call "Send to Consumer.vi"("error in (no error)"=w990, "Case ID"=Monkey_Consumer_Case_Selector."Update GUI" ("Monkey Consumer Case Selector"), "uService Template in"=w992) -> ("error out"=w995:errorcluster, "uService Template out"=w997:refnum<class "Monkey.lvclass">)  [unwired: 7 in]
        }
        frame "Delete cell" {
          n310 = in-place {
            n311 = in-place-cluster #3(w1006) -> ("Run block"=w1009:refnum<class "Run Block.lvclass">)
            n312 = call-dynamic "Delete Cell.vi"("Run Block in"=w1009) -> ("Run Block out"=w1008:refnum<class "Run Block.lvclass">)  [unwired: 9 in, 1 out]
            n313 = in-place-cluster #3("Run block"=w1008) -> (w1003:refnum<class "Monkey.lvclass">)
          }
          n314 = call "Send to Consumer.vi"("error in (no error)"=w1005, "Case ID"=Monkey_Consumer_Case_Selector."Update GUI" ("Monkey Consumer Case Selector"), "uService Template in"=w1003) -> ("error out"=w1004:errorcluster, "uService Template out"=w1002:refnum<class "Monkey.lvclass">)  [unwired: 7 in]
        }
        frame "Move cell" {
          n315 = Variant To Data(type=TRUE, Variant=w1012) -> (data=w1010:bool)  [unwired: 1 in, 1 out]
          n316 = in-place {
            in-place-border: w1010 -> [w1019]
            n317 = in-place-cluster #4(w1017) -> ("Run block"=w1021:refnum<class "Run Block.lvclass">)
            n318 = call-dynamic "Move Cell.vi"("Up/Down"=w1019, "Run Block in"=w1021) -> ("Run Block out"=w1020:refnum<class "Run Block.lvclass">)  [unwired: 8 in, 1 out]
            n319 = in-place-cluster #4("Run block"=w1020) -> (w1014:refnum<class "Monkey.lvclass">)
          }
          n320 = call "Send to Consumer.vi"("error in (no error)"=w1016, "Case ID"=Monkey_Consumer_Case_Selector."Update GUI" ("Monkey Consumer Case Selector"), "uService Template in"=w1014) -> ("error out"=w1015:errorcluster, "uService Template out"=w1013:refnum<class "Monkey.lvclass">)  [unwired: 7 in]
        }
      }
    }
    frame Error {
    }
  }
  n321 = call-parent "Consumer.vi"("error in (no error)"=w6, "Data"="Data", "Case ID"="Case ID", "uService Template in"=w3) -> ("error out"=→"error out":errorcluster, "uService Template out"=→"Monkey out":refnum<class "Monkey.lvclass">)  [unwired: 6 in]
